vi "DialogCreateClass.vi"(0 "ClassWriterNative.lvclass":refnum<class "ClassWriterNative.lvclass">, 1 "ProjectItem Refnum":refnum<vi>, 5 "error in (no error)":errorcluster) -> (13 "InterfaceToImplement":T5, 14 "Reference out":refnum<class "ClassWriterNative.lvclass">, 15 "Cancelled":bool, 16 "CreateClassData":T6, 17 "DesignPatternsToAddAfterCreation":string[](array[string]), 18 "ChangeProviderRequested":string, 19 "error out":errorcluster)   [LabVIEW 2020, in "ClassWriterNative.lvclass"]
uses:
  <resource>/Framework/Providers/Open_GDS/ClassProviders/Provider_LvNativeClass/ClassWriterNative_class/ClassWriterNative.lvclass
  C:/Program Files (x86)/National Instruments/LabVIEW 2020/resource/Framework/Providers/Open_GDS/ClassProviders/Provider_BaseClassInterface/ClassWriter_class/ClassWriter.lvclass
  <resource>/Framework/Providers/Open_GDS/ClassProviders/Provider_BaseClassInterface/CreateClassData.ctl
  <resource>/Framework/Providers/Open_GDS/ClassProviders/Provider_BaseClassInterface/ClassWriter_class/InterfacesToImplement.ctl
  <resource>/Framework/Providers/Open_GDS/ClassProviders/Common/ScriptingFunctions/Scripting_ConnectorPanePatternType.ctl
  <resource>/Framework/Providers/Open_GDS/ClassProviders/Provider_BaseClassInterface/BaseProvider_SubVIs/BaseProvider_WireList.ctl
  <resource>/Framework/Providers/Open_GDS/ClassProviders/Provider_BaseClassInterface/BaseProvider_SubVIs/BaseProvider_WireStyleType.ctl
  <resource>/Framework/Providers/Open_GDS/ClassProviders/Provider_BaseClassInterface/ClassTemplateType.ctl
  <resource>/Framework/Providers/Open_GDS/ClassProviders/Common/InterfaceLibrary/InterfaceInfo.ctl
  <resource>/Framework/Providers/Open_GDS/ClassProviders/Common/LvClass_class/GDSLvClass_ClassMethodInfo.ctl
  <vilib>/Utility/miscctls.llb/LVRectTypeDef.ctl
  <vilib>/Utility/miscctls.llb/LVPositionTypeDef.ctl
  <resource>/Framework/Providers/Open_GDS/ClassProviders/Provider_EndevoGOOP400/EndevoG4ProviderName.ctl
  <vilib>/Utility/miscctls.llb/LVPointTypeDef.ctl
  <vilib>/Utility/miscctls.llb/LVNodeAndColumnTypeDef.ctl
  <vilib>/picture/picture.llb/imagedata.ctl
  <vilib>/Utility/miscctls.llb/LVRowAndColumnUnsignedTypeDef.ctl
  5375c306-5cef-40a8-bf77-a54f91188c9c.vi
  <resource>/Framework/Providers/Open_GDS/ClassProviders/Provider_BaseClassInterface/ClassWriter_class/ClassWriter.lvclass
  <resource>/Framework/Providers/Open_GDS/ClassProviders/Common/InterfaceLibrary/InterfaceLibrary.lvlib
panel:
  in  "WireSelectionList":T1
  out "IconSelection":picture
  in  "ModifyProviders":bool
  in  "Help":bool
  in  "_ShowContextHelp":bool
  out "Icon":picture
  in  "ConnectorPanePattern":T3 caption="Connector Pane" items=["4x4x4", "5x6x5", "6x8x6"]
  in  "ModifyTemplates":bool
  in  "AddDesignPattern":bool caption="DESIGN PATTERN"
  out "ProductPicture":picture
  out "TriggerSuffixChange":string
  in  "_CurrentClassProvider":u16(ring) caption="Class Provider To Use" items=["By Reference DVR (GOOP4)", "LVClass by value", "By Reference (GOOP3)"]
  in  "_UseLLB":bool
  out "DupPath":bool
  in  "_ClassType":i32(listbox) caption="Class Templates"
  in  "_ClassFolderSuffix":string caption="Folder Suffix"
  in  "_ClassName":string caption="Class Name"
  in  "_ClassDescription":string caption="Class Description"
  in  "_ClassFolder":path caption="Save Class To.."
  out "Wire Style":cluster{"Name":string, "Wire":picture}
  in  "ParentClassFilter":string caption="Filter"
  in  "_SelectParentClass":string(tree)="Derived Class" caption="Select Parent Class"
  in  "CreateInterfaceMethods":T4(ring)
  in  "InterfaceFilter":string caption="Filter"
  in  "_SelectInterfaceClass":i32[](listbox) caption="Select Parent Interface(s) (ctrl+click to do multiple Selection)"
  in  "_Cancel":bool
  in  "_CreateClass":bool
  out "DesignPatternDescription":string caption="Design Pattern Description"
  in  "DesignPatternList":i32(listbox) caption="Design Patterns"
  # "DESIGN PATTERNS SELECTION"
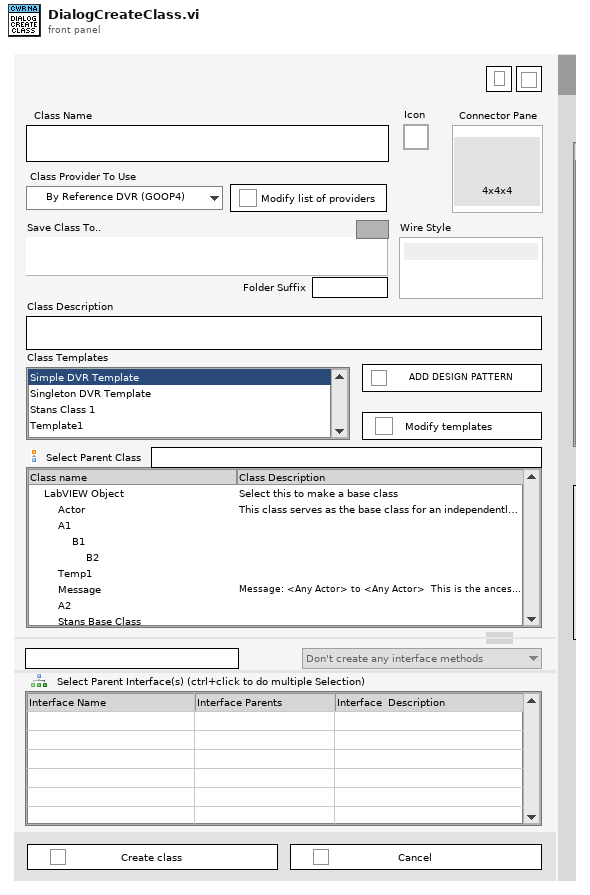
[diagram p1: front panel]
types:
  T1 = typedef "BaseProvider_WireList.ctl" = cluster{"WireStyle":T2[], "WireEditor":bool}
  T2 = typedef "BaseProvider_WireStyleType.ctl" = cluster{"Boolean":bool, "Wire":picture, "Name":string, "Status":u16}
  T3 = typedef "Scripting_ConnectorPanePatternType.ctl" = u16
  T4 = enum16{"Don't create any interface methods", "Create some interface methods", "Create all interface methods"}
  T5 = typedef "ClassWriter.lvclass/InterfacesToImplement.ctl" = cluster{"InterfacePath":path[], "CreateMethods":bool, "MethodsPerInterface(Empty=>All)":cluster{"Methods":string[]}[]}
  T6 = typedef "ClassWriter.lvclass/CreateClassData.ctl" = cluster{"ClassName":string, "ClassFolder":path, "ClassDescription":string, "ClassTemplateOptions":string, "BaseClass(ProjectStringPath or LvClassFilePath)":variant, "ExtraCreateParameters":variant, "FolderSuffix":string, "ParentInterfaces":path[]}
  T7 = cluster{"Font Name":string, "Size":u16, "Bold":bool, "Italic":bool, "Underline":bool, "Strikeout":bool, "Color":u32}
  T8 = typedef "LVPositionTypeDef.ctl" = cluster{"Left":i32, "Top":i32}
  T9 = typedef "LVRectTypeDef.ctl" = cluster{"Left":i16, "Top":i16, "Right":i16, "Bottom":i16}
  T10 = typedef "ClassWriter.lvclass/ClassTemplateType.ctl" = cluster{"TemplateIdName":string, "TemplateUserDialogName":string, "OnlySubClassTemplate":bool, "CanDeriveFromTheseTemplateIDs":string[], "ClassSuffix":string, "Description":string, "LvLibTemplate":bool, "CustomLocation":path}
  T11 = typedef "InterfaceLibrary.lvlib/InterfaceInfo.ctl" = cluster{"Name(Short if no Conflicts)":string, "FullQualifierName":string, "Description":string, "Path":path, "ParentInterfaceNames(Short if no Conflitcs)":string[], "ParentInterfaceFullQualifierNames":string[], "IconPath":path, "Methods":T12[], "DynamicDispatchMethod":bool[]}
  T12 = typedef "GDSLvClass_ClassMethodInfo.ctl" = cluster{"Name":string, "Descriptions":string, "RelativePath":path, "SourceScope":enum32{"invalid scope", "public", "private", "protected", "community"}, "MustOverride":bool, "VirtualFolderLocation":string[], "DynamicDispatch":bool}
  T13 = cluster{"Cancel":bool, "OtherTemplates":string[], "BaseClasses":path[], "Templates":T10[], "BaseObjectTag":string, "ClassType(Template)":string, "BaseClassToUse":path, "DeriveFromClass":path, "OpenG":bool, "Derived":bool, "DeriveFromClassRef":refnum<vi>, "ClassPaths":path[], "DesignPatternsVisible":bool, "ClassProviderName":string, "ClassTemplateUsed":string, "PlugInIDs":string[], "DPDescriptions":string[], "DpDependencies":cluster{"DependenciesID":string[]}[], "DPs":string[], "InitDerived":bool, "ClassFolderSuffix":string, "ChangeProviderTo":string, "ClassTags":string[], "LLB_Allowed":bool, "StartFolder":path, "SplitterMouseDown":bool, "InterfaceIcons":path[], "InterfaceInfo":T11[], "OldBnds":T9, "BondsChanged":bool, "ClassTemplateIndex":i32[], "StartBnds":T9, "StartInterfacePath":path, "Providers":string[], "LastProvderValues":cluster{"_ClassName":string, "_ClassFolder":path, "_ClassDescription":string, "Created":timestamp}, "ParentInterfaces":path[], "InterfacesInList":path[]}
  T14 = typedef "EndevoG4ProviderName.ctl" = enum16{"EndevoGOOP400"}
  T15 = typedef "LVPointTypeDef.ctl" = cluster{"Horizontal":i16, "Vertical":i16}
  T16 = typedef "LVNodeAndColumnTypeDef.ctl" = cluster{"Node":string, "Column":i32}
  T17 = typedef "imagedata.ctl" = cluster{"image type":i32, "image depth":i32, "image":u8[], "mask":u8[], "colors":u32[], "Rectangle":cluster{"left":i16, "top":i16, "right":i16, "bottom":i16}}
  T18 = typedef "LVRowAndColumnUnsignedTypeDef.ctl" = cluster{"Row":u32, "Column":u32}
  T19 = enum8{"Enabled", "Disabled", "Disabled and Grayed Out"}
  T20 = cluster{"_ClassName":string, "_ClassFolder":path, "_ClassDescription":string, "seconds since 1Jan1904":timestamp}
  T21 = typedef "GDSLvCLass_ClassSettingsType.ctl" = cluster{"ClassProviderName":string, "ClassTemplateUsed":string, "ClassTemplateVersion":string, "ClassDescription":string, "PlugIns":T22[], "ConnectorPanePattern":string}
  T22 = typedef "GDSLvClass_PlugIn.ctl" = cluster{"Type":T23, "ID":string, "Version":string, "Path":path, "Name":string, "Data":variant}
  T23 = typedef "GDSLvClass_PlugInTypes.ctl" = enum16{"DesignPattern", "MethodTypes"}
  T24 = typedef "BaseProvider_IniFileSettings.ctl" = cluster{"ClassFolderSuffix":string, "InterfaceFolderSuffix":string, "InterfaceIcon":string, "FileNamingOption":T25, "DynamicDispatchStartValue":bool, "UseGetSetForPropertyNodeMethods":bool}
  T25 = typedef "BaseProvider_FileNamingOption.ctl" = enum16{"CamelCase", "Space", "Underscore"}
  T26 = enum32{"Invalid", "Standard", "Closed", "Hidden", "Minimized", "Maximized"}
  T27 = cluster{"_ClassName":string, "_ClassFolder":path, "_ClassDescription":string, "Created":timestamp}
  T28 = typedef "GOOP_WireConfigurationType.ctl" = cluster{"Edge thickness":i32, "Edge color":u32, "Center thickness":i32, "Center pattern":T29, "CenterColor1":u32, "CenterColor2":u32, "Tunnels and terminals colors":u32}
  T29 = typedef "GOOP_WirePattern.ctl" = enum16{"Solid", "Large dash", "Small dash"}
  T30 = typedef "LVPoint32TypeDef.ctl" = cluster{"Horizontal":i32, "Vertical":i32}
  T31 = typedef "DesignPatternsData.ctl" = cluster{"Type":string, "Patterns":cluster{"ID":string, "Path":path, "Name":string, "Desc":string, "Version":string, "DependenciesID":string[], "OnlyOne":bool}[]}
  T32 = cluster{"ID":string, "Path":path, "Name":string, "Desc":string, "Version":string, "DependenciesID":string[], "OnlyOne":bool}[]
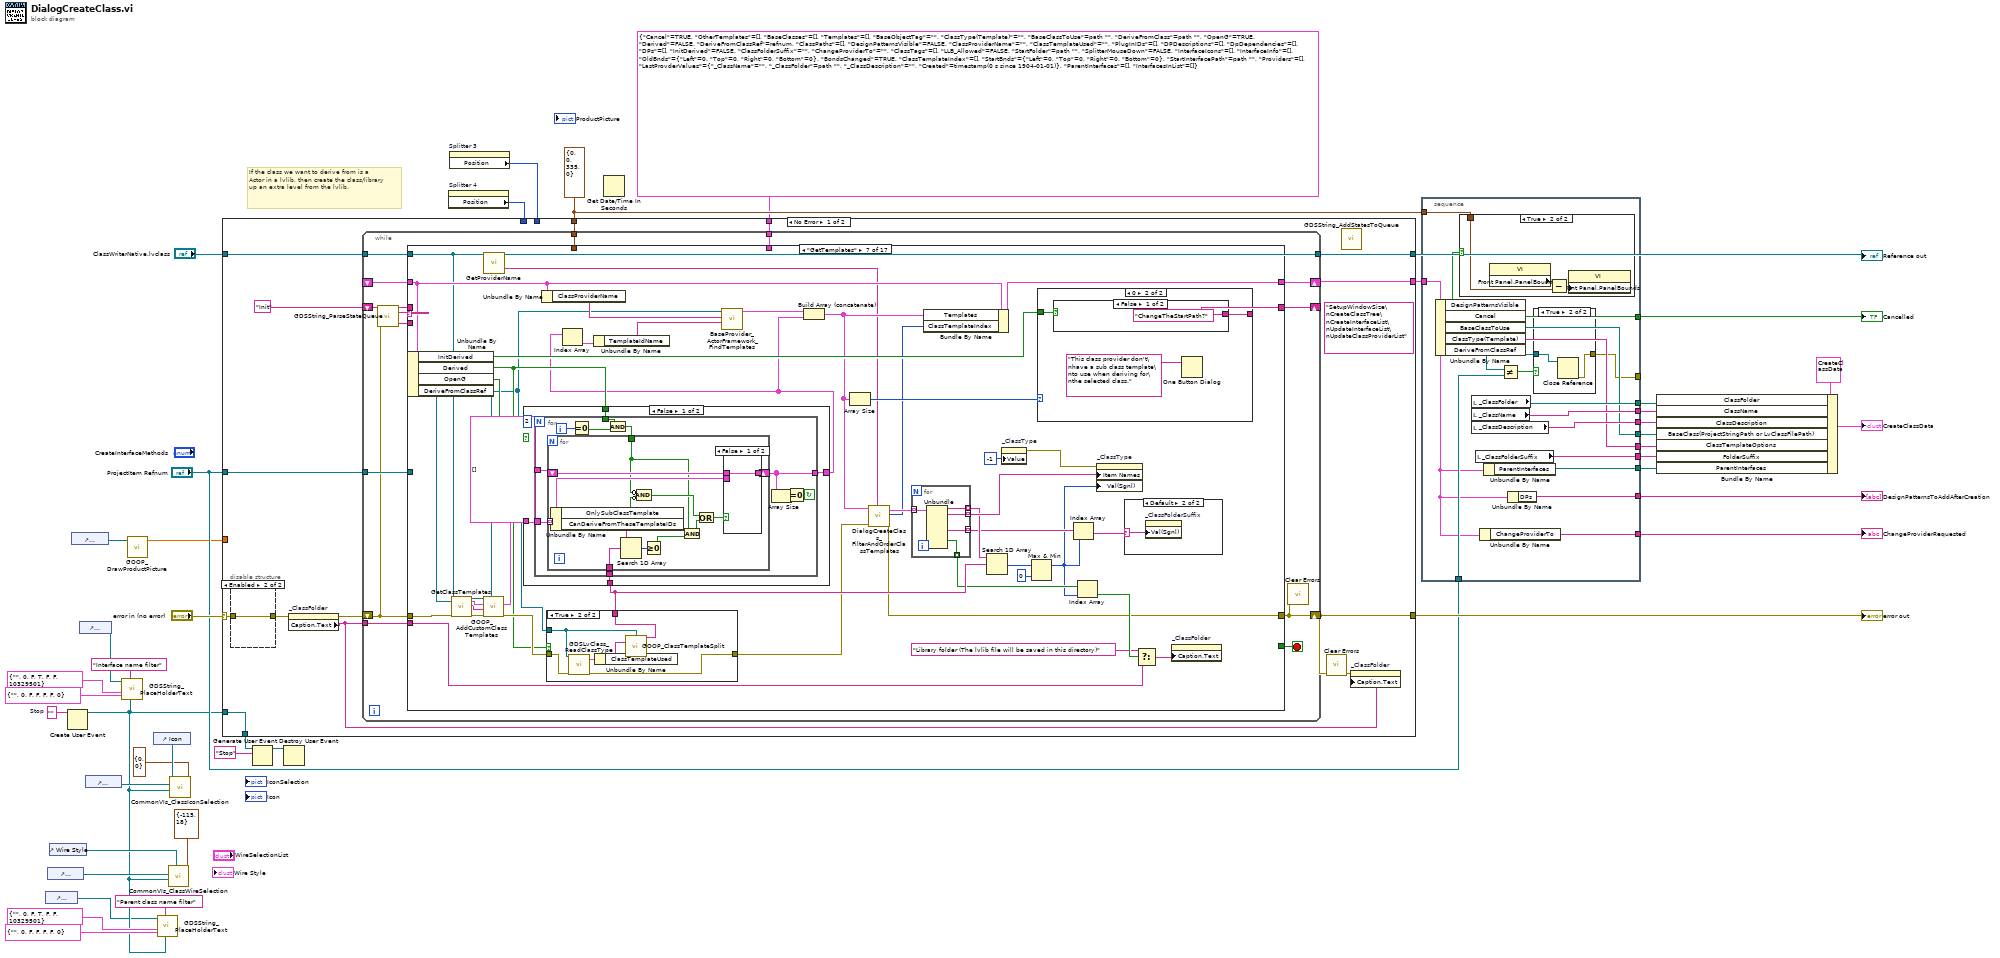
[diagram p0: block diagram]
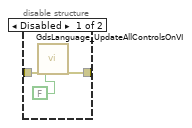
[diagram p4: hidden frame]
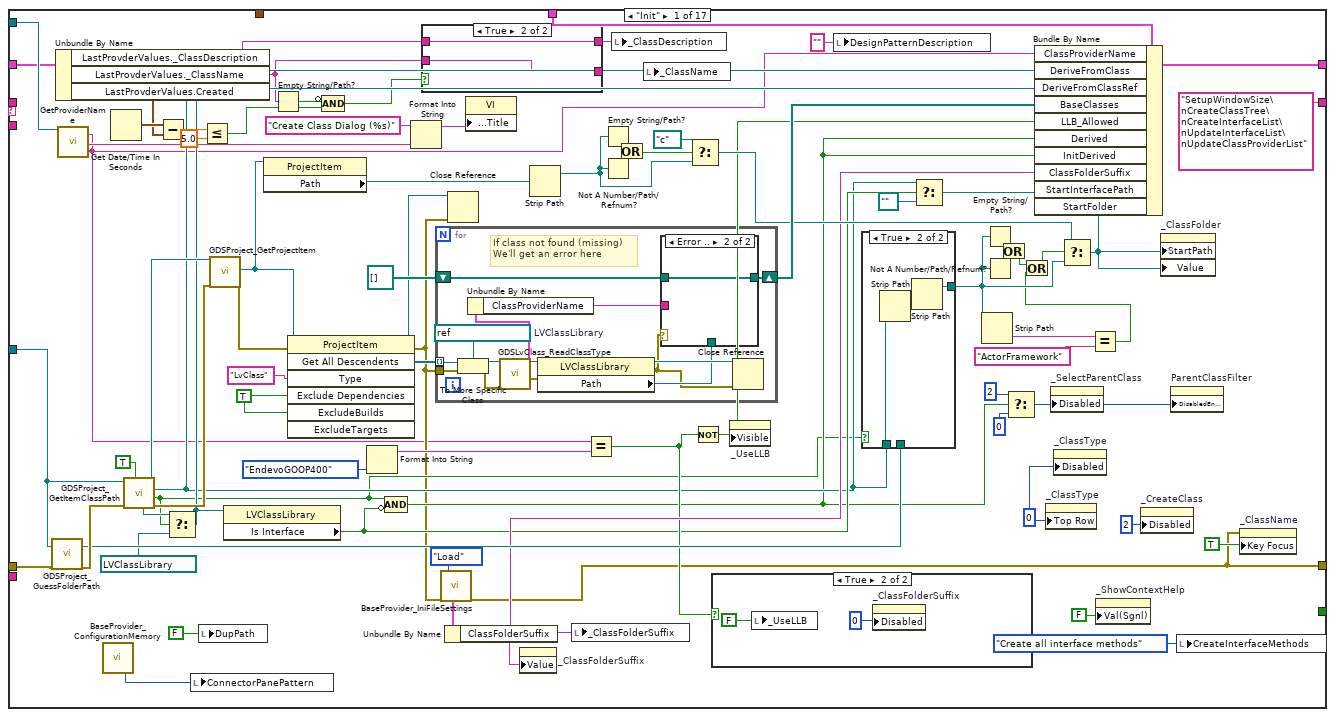
[diagram p5: hidden frame]
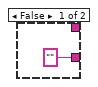
[diagram p6: hidden frame]
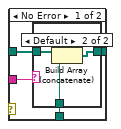
[diagram p8: hidden frame]
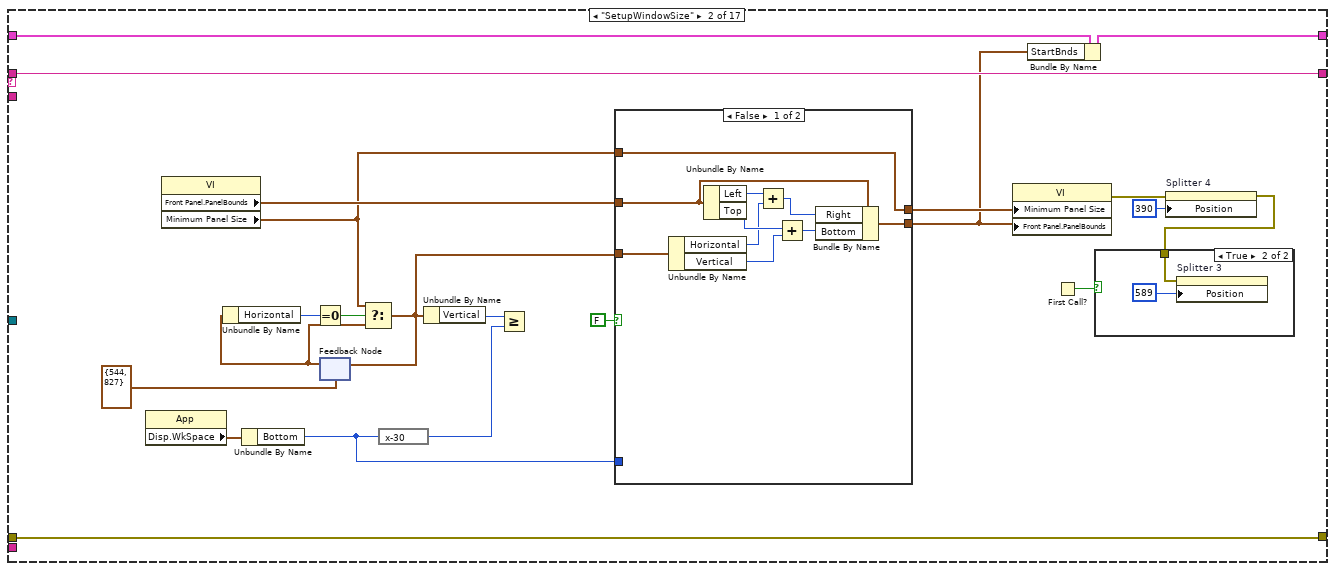
[diagram p11: hidden frame]
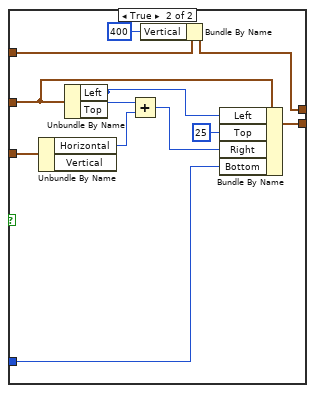
[diagram p13: hidden frame]
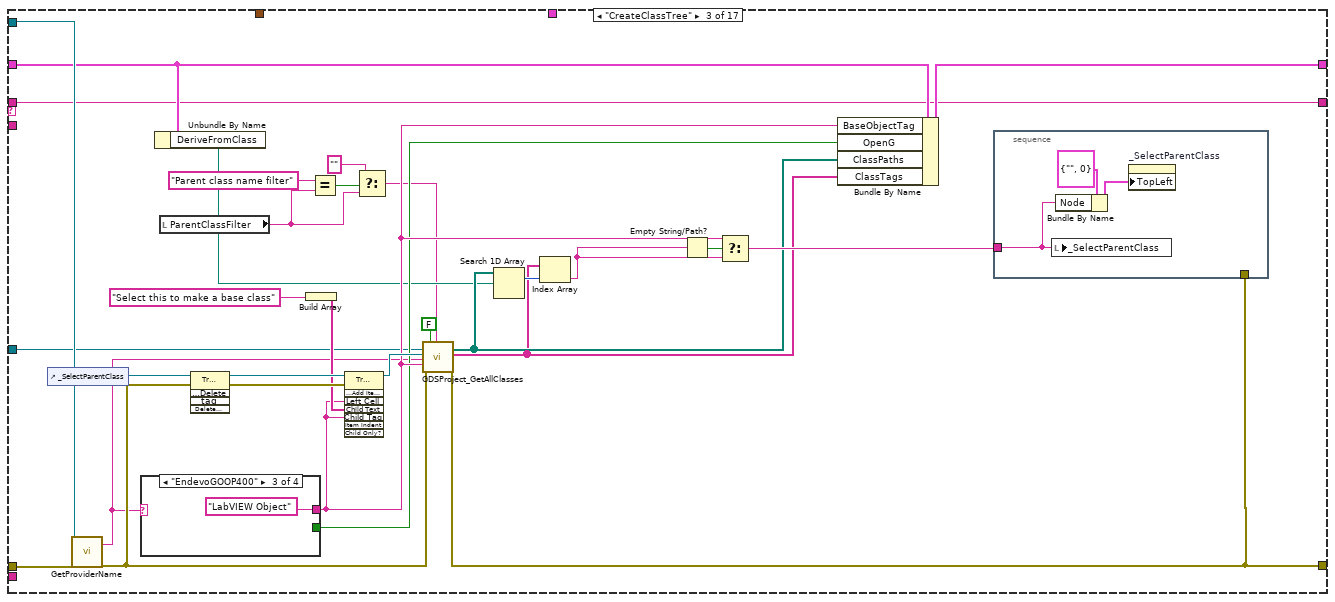
[diagram p14: hidden frame]
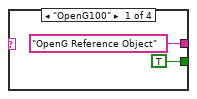
[diagram p15: hidden frame]
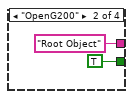
[diagram p16: hidden frame]
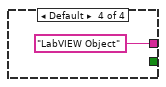
[diagram p17: hidden frame]
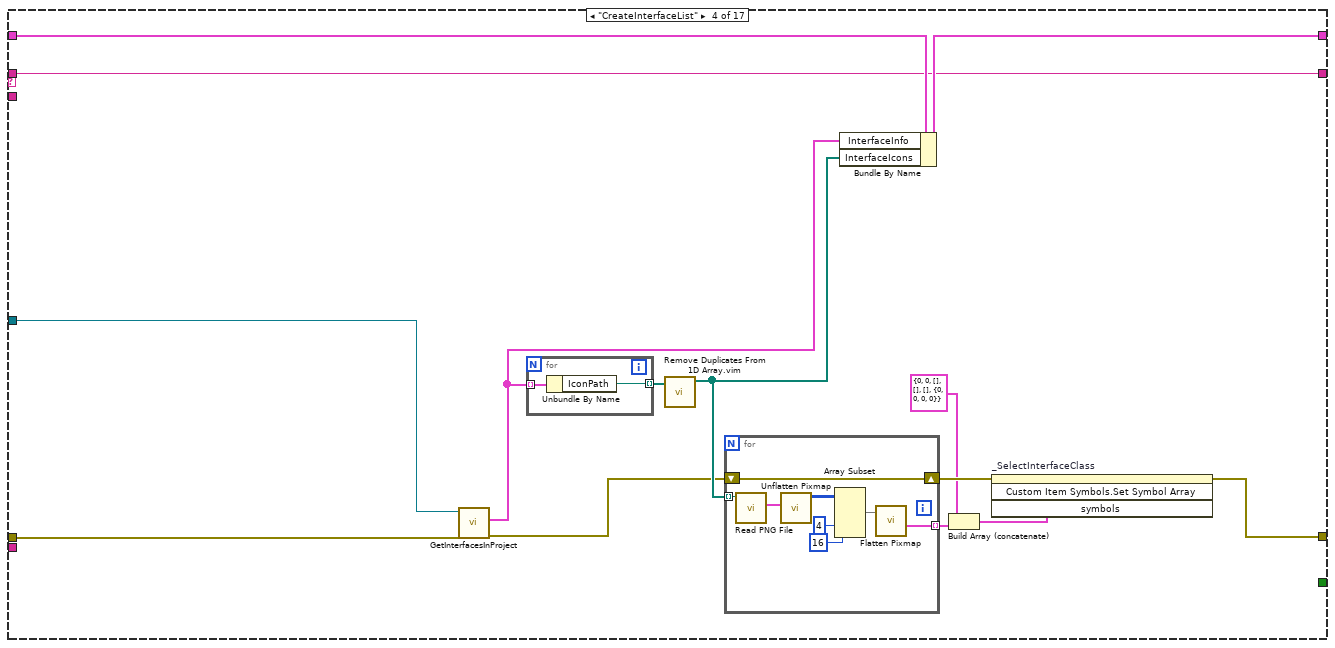
[diagram p18: hidden frame]
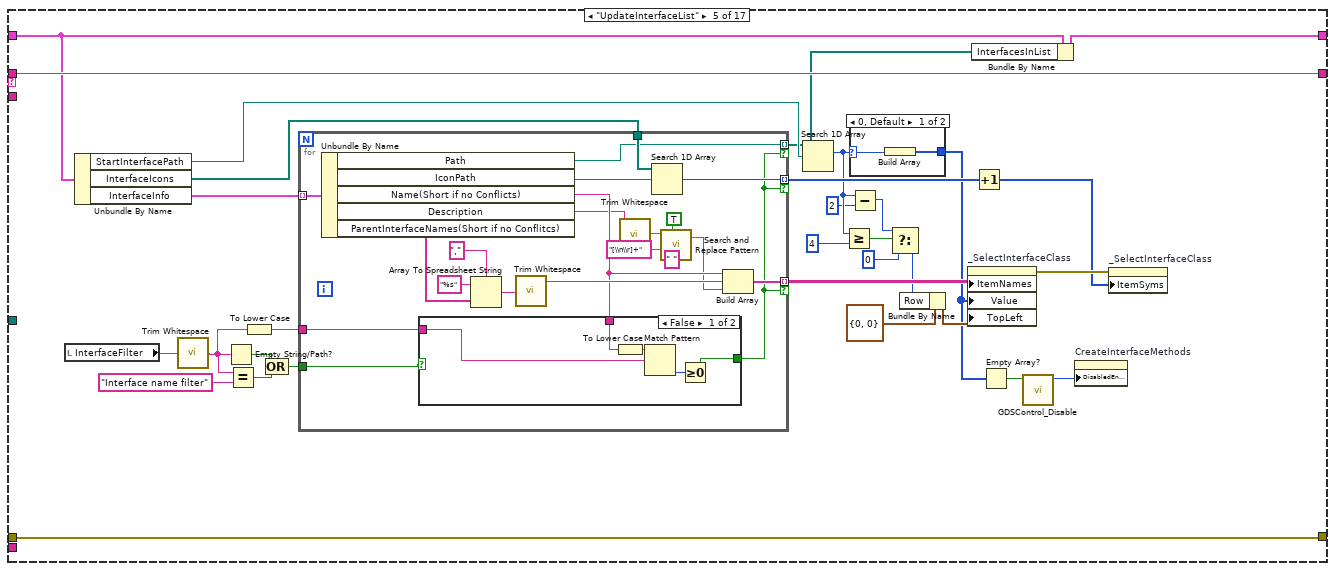
[diagram p19: hidden frame]
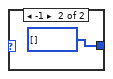
[diagram p20: hidden frame]
diagram:
  w16 = ""  # Stop
  w29 = T9 {"Left"=0, "Top"=0, "Right"=335, "Bottom"=0} ("Rect")
  # "If the class we want to derive from is a\nActor in a lvlib, then create the class/library\nup an extra level from the lvlib."
  n1 = control-ref of="ParentClassFilter"() -> (w1:refnum<vi>)
  n2 = control-ref of="WireSelectionList"() -> (w10:refnum<vi>)
  n3 = control-ref of="Wire Style"() -> (w9:refnum<vi>)
  n4 = Create User Event(user event datatype=w16) -> (user event=w2:refnum<user-event>)  [unwired: 1 in, 1 out]
  n5 = control-ref of="ProductPicture"() -> (w25:refnum<vi>)
  n6 = control-ref of="InterfaceFilter"() -> (w23:refnum<vi>)
  n7 = control-ref of="IconSelection"() -> (w17:refnum<vi>)
  n8 = call <resource>:"GDSString_PlaceHolderText.vi"("BooleanUserEventToStopPlaceHolderVI"=w2, "PlaceholderText"="Interface name filter" ("InterfaceFilter"), "PlaceholderTextFont(Grey,Italic)"=T7 {"Font Name"="", "Size"=0, "Bold"=FALSE, "Italic"=TRUE, "Underline"=FALSE, "Strikeout"=FALSE, "Color"=10329501}, "NormalTextFont(Black)"=T7 {"Font Name"="", "Size"=0, "Bold"=FALSE, "Italic"=FALSE, "Underline"=FALSE, "Strikeout"=FALSE, "Color"=0}, "PlaceholderStringRef"=w23) -> ()  [unwired: 6 in, 1 out]
  n9 = call <resource>:"GOOP_DrawProductPicture.vi"("ProductPictureControl"=w25) -> ("Zoom Factor"=w24:sgl)  [unwired: 10 in]
  n10 = control-ref of="Icon"() -> (w18:refnum<vi>)
  n11 = call <resource>:"GDSString_PlaceHolderText.vi"("BooleanUserEventToStopPlaceHolderVI"=w2, "PlaceholderText"="Parent class name filter" ("InterfaceFilter"), "PlaceholderTextFont(Grey,Italic)"=T7 {"Font Name"="", "Size"=0, "Bold"=FALSE, "Italic"=TRUE, "Underline"=FALSE, "Strikeout"=FALSE, "Color"=10329501}, "NormalTextFont(Black)"=T7 {"Font Name"="", "Size"=0, "Bold"=FALSE, "Italic"=FALSE, "Underline"=FALSE, "Strikeout"=FALSE, "Color"=0}, "PlaceholderStringRef"=w1) -> ()  [unwired: 6 in, 1 out]
  n12 = call <resource>:"CommonVIs_ClassWireSelection.vi"("Offset(-300,0)"=T8 {"Left"=-115, "Top"=18}, "SelectedWireStyle"=w9, "Messages(Stop or Empty string will stop this VI)"=w2, "WireSelectionList"=w10) -> ()  [unwired: 7 in, 1 out]
  n13 = call <resource>:"CommonVIs_ClassIconSelection.vi"("Offset"=T8 {"Left"=0, "Top"=0}, "Icon"=w18, "Messages(Stop or Empty string will stop this VI)"=w2, "IconSelection"=w17) -> ()  [unwired: 8 in]
  n14 = property on="Splitter 4" class="Splitter"() -> ("Position"=w13:i32)  [unwired: 2 in, 2 out]
  n15 = property on="Splitter 3" class="Splitter"() -> ("Position"=w12:i32)  [unwired: 2 in, 2 out]
  n16 = case shown="No Error" "error in (no error)" {
    selector: "error in (no error)" -> [w52 w1129]
    tunnel: "ClassWriterNative.lvclass" -> [w56 w1128]
    tunnel: [w45 w1129] -> w42
    tunnel: [w57 w1128] -> w40
    tunnel: T13 {"Cancel"=TRUE, "OtherTemplates"=[], "BaseClasses"=[], "Templates"=[], "BaseObjectTag"="", "ClassType(Template)"="", "BaseClassToUse"=path "", "DeriveFromClass"=path "", "OpenG"=TRUE, "Derived"=FALSE, "DeriveFromClassRef"=refnum, "ClassPaths"=[], "DesignPatternsVisible"=FALSE, "ClassProviderName"="", "ClassTemplateUsed"="", "PlugInIDs"=[], "DPDescriptions"=[], "DpDependencies"=[], "DPs"=[], "InitDerived"=FALSE, "ClassFolderSuffix"="", "ChangeProviderTo"="", "ClassTags"=[], "LLB_Allowed"=FALSE, "StartFolder"=path "", "SplitterMouseDown"=FALSE, "InterfaceIcons"=[], "InterfaceInfo"=[], "OldBnds"={"Left"=0, "Top"=0, "Right"=0, "Bottom"=0}, "BondsChanged"=TRUE, "ClassTemplateIndex"=[], "StartBnds"={"Left"=0, "Top"=0, "Right"=0, "Bottom"=0}, "StartInterfacePath"=path "", "Providers"=[], "LastProvderValues"={"_ClassName"="", "_ClassFolder"=path "", "_ClassDescription"="", "Created"=timestamp(0 s since 1904-01-01)}, "ParentInterfaces"=[], "InterfacesInList"=[]} ("output cluster") -> [w55 _]
    tunnel: "ProjectItem Refnum" -> [w54 _]
    tunnel: [w53 _] -> w39
    tunnel: w29 -> [w51 _]
    tunnel: w24 -> [_ _]
    tunnel: w2 -> [w47 w1127]
    tunnel: [w47 w1127] -> w20
    tunnel: w13 -> [_ _]
    tunnel: w12 -> [_ _]
    frame No Error {
      (unwired) "SetupWindowSize\nCreateClassTree\nCreateInterfaceList\nUpdateInterfaceList\nUpdateClassProviderList"
      n17 = disable-structure shown="Enabled" {
        disable-tunnel: w52 -> [w60 w61]
        disable-tunnel: [w58 w61] -> w50
        frame Disabled {
          n18 = call <resource>:"GdsLanguage_UpdateAllControlsOnVI.vi"("error in (no error)"=w60, "CreateLanguageFile(Use this to create a languageFile)"=FALSE) -> ("error out"=w58:errorcluster)  [unwired: 16 in, 1 out]
        }
        frame Enabled {
        }
      }
      n19 = property on="_ClassFolder" class="Path"(error in=w50) -> (error out=w49:errorcluster, "Caption.Text"=w48:string)  [unwired: 1 in, 1 out]
      n20 = while {
        shift-right: [w62] -> w45
        shift-left: w49 -> [w68]
        shift-right: [w66] -> _
        shift-left: "Init" -> [w69]
        shift-right: [w72] -> w53
        shift-left: _ -> [w76]
        tunnel: w56 -> [w75]
        tunnel: [w75] -> w57
        tunnel: w55 -> [w74]
        tunnel: w54 -> [w73]
        tunnel: w51 -> [w71]
        tunnel: w48 -> [w70]
        stop <- w67 stop-if-true
        n21 = call <resource>:"GDSString_ParseStateQueue.vi"("State Queue"=w69, "Error In (no error)"=w68) -> ("Remaining States"=w64:string, "Current State"=w65:string, "Arguments"=w63:string)  [unwired: 9 in, 2 out]
        n22 = case shown="\"GetTemplates\"" w65 {
          tunnel: w76 -> [w92 w209 w253 w284 w324 w366 w405 w483 w509 w518 w914 w928 w957 w1018 w1096 w1122 w1126]
          tunnel: [w154 w193 w255 w285 w300 w365 w421 w483 w509 w538 w915 w943 w956 w1045 w1096 w1122 w1126] -> w72
          tunnel: w68 -> [w134 w208 w258 w272 w325 w372 w418 w479 w508 w541 w919 w945 w966 w1036 w1102 _ w1125]
          tunnel: [w80 w208 w238 w276 w325 w372 w390 w479 w508 w541 w919 w945 w965 w1035 w1102 errorcluster {"status"=TRUE, "code"=1, "source"="Invalid Case"} ("error out") w1125] -> w62
          tunnel: w75 -> [w127 _ w261 _ _ w367 w383 _ _ w511 _ w921 _ _ _ _ _]
          tunnel: ["SetupWindowSize\nCreateClassTree\nCreateInterfaceList\nUpdateInterfaceList\nUpdateClassProviderList" w207 w239 w273 w326 "GetTemplates" w422 "Idle" "Idle" w539 w918 w944 "Idle" "GetInterfaceSettings" "Exit" "Exit" "Exit"] -> w66
          tunnel: w74 -> [w153 _ _ _ _ _ _ _ _ _ _ _ _ _ _ _ _]
          tunnel: w73 -> [w132 _ w240 w283 _ _ _ _ _ w523 _ _ _ _ _ _ _]
          tunnel: w71 -> [_ _ _ _ _ _ _ _ _ w521 _ _ _ _ _ _ _]
          tunnel: w70 -> [_ _ _ _ _ _ w398 _ _ w520 _ w930 _ _ _ _ _]
          tunnel: [_ _ _ _ _ _ _ _ _ _ _ _ _ _ _ TRUE TRUE] -> w67
          tunnel: w64 -> [_ w207 w239 w273 w326 _ _ _ _ _ w918 w944 _ _ _ _ _]
          tunnel: w63 -> [_ _ _ _ _ _ _ _ _ _ _ _ _ _ _ _ _]
          frame "Init" {
            w123 = 0 ("Top Row")
            w126 = TRUE ("ExcludeDependencies")
            n23 = call <resource>:"GDSProject_GuessFolderPath.vi"("ProjectItem"=w132, "error in (no error)"=w134) -> ("Path"=w131:path, "error out"=w133:errorcluster)  [unwired: 14 in, 2 out]
            n24 = Unbundle By Name(w92) -> ("LastProvderValues._ClassDescription"=w84:string, "LastProvderValues._ClassName"=w85:string, "LastProvderValues.Created"=w90:timestamp)
            n25 = call-dynamic "GetProviderName.vi"("ClassWriterNative in"=w127) -> ("ProviderName"=w78:string, "TranslatedProviderName"=w79:string)  [unwired: 14 in, 3 out]
            n26 = call <resource>:"BaseProvider_ConfigurationMemory.vi"() -> ("PatternOut"=w103:T3)  [unwired: 13 in, 6 out]
            n27 = Get Date/Time In Seconds() -> (seconds since 1Jan1904=w91:timestamp)
            n28 = call <resource>:"GDSProject_GetItemClassPath.vi"("ReturnRefToClass(False)"=TRUE, "error in"=w133, "ProjectItemRefIn"=w132) -> ("error out"=w150:errorcluster, "LvCLassFound"=w93:bool, "Path"=w99:path, "ProjectItemRefOut"=w148:refnum<vi>, "LvClassRef"=w122:refnum<vi>)  [unwired: 3 in, 1 out]
            n29 = Subtract(x=w91, y=w90) -> (x-y=w89:dbl)
            n30 = Select(t=w122, s=w93, f=refnum<vi> refnum) -> (s? t:f=w101:refnum<vi>)
            n31 = local write "ConnectorPanePattern"(w103) -> ()
            n32 = local write "DupPath"(FALSE ("DupPath")) -> ()
            n33 = Less Or Equal?(x=w89, y=5.0) -> (x <= y?=w86:bool)
            n34 = call <resource>:"GDSProject_GetProjectItem.vi"("ProjectItemToSearchFrom"=w148, "error in (no error)"=w150) -> ("ProjectItemFound"=w102:refnum<vi>, "error out"=w149:errorcluster)  [unwired: 14 in, 2 out]
            n35 = property class="LVClassLibrary"(reference=w101) -> ("Is Interface"=w100:bool)  [unwired: 1 in, 2 out]
            n36 = property class="ProjectItem"(reference=w102) -> ("Path"=w136:path)  [unwired: 1 in, 2 out]
            n37 = Empty String/Path?(string/path=w85) -> (empty?=w87:bool)
            n38 = invoke class="ProjectItem" method="Get All Descendents"(reference=w102, error in=w149, "Type"="LvClass" ("x"), "Exclude Dependencies"=w126, "ExcludeBuilds"=w126) -> (reference out=w145:refnum<vi>, error out=w80:errorcluster, "All Descendents"=w147:refnum<vi>[])  [unwired: 2 in, 4 out]
            n39 = Compound Arithmetic op=AND(invert w87, w86) -> (w83:bool)
            n40 = Format Into String(EndevoG4ProviderName."EndevoGOOP400" ("ProviderName")) -> (resulting string=w118:string)  [unwired: 3 in, 1 out]
            n41 = Compound Arithmetic op=AND(w93, invert w100) -> (w96:bool)
            n42 = Format Into String(format string="Create Class Dialog (%s)", w79) -> (resulting string=w129:string)  [unwired: 2 in, 1 out]
            n43 = case shown="True" w83 {
              tunnel: w85 -> [_ w157]
              tunnel: w84 -> [_ w158]
              tunnel: [_ w158] -> w82
              tunnel: ["" ("Class name") w157] -> w81
              frame False {
              }
              frame True {
              }
            }
            n44 = for {
              tunnel: w147 -> [w174] mode=indexing
              shift-right: [w170] -> w144
              shift-left: path[] [] -> [w169]
              tunnel: w80 -> [w166]
              w173 = refnum<vi> refnum  # LVClassLibrary
              # "If class not found (missing)\nWe'll get an error here"
              n45 = To More Specific Class(target class=w173, reference=w174, error in=w166) -> (specific class reference=w172:refnum<vi>, error out=w171:errorcluster)
              n46 = call <resource>:"GDSLvClass_ReadClassType.vi"("Class Refnum In"=w172, "error in (no error)"=w171) -> ("Class Refnum Out"=w167:refnum<vi>, "ClassSettings"=w165:T21, "error out"=w168:errorcluster)  [unwired: 15 in]
              n47 = Unbundle By Name(w165) -> ("ClassProviderName"=w164:string)
              n48 = property class="LVClassLibrary"(reference=w167, error in=w168) -> (reference out=w163:refnum<vi>, error out=w161:errorcluster, "Path"=w162:path)
              n49 = case shown="Error .." w161 {
                tunnel: [w178 w183] -> w170
                tunnel: w169 -> [w177 w183]
                tunnel: w164 -> [w176 _]
                tunnel: w162 -> [w175 _]
                frame No Error {
                  n50 = case shown="Default" w176 {
                    tunnel: [w179 w182] -> w178
                    tunnel: w177 -> [w179 w181]
                    tunnel: w175 -> [_ w180]
                    frame "" {
                    }
                    frame Default {
                      n51 = Build Array (concatenate)(w181, w180) -> (w182:path[])
                    }
                  }
                }
                frame Error {
                }
              }
              n52 = Close Reference(reference=w163, error in (no error)=w161) -> ()  [unwired: 1 out]
            }
            n53 = call <resource>:"BaseProvider_IniFileSettings.vi"("error in (no error)"=w80, "Action"=enum16{"Read", "Load", "Save"}."Load") -> ("IniFileSettings"=w116:T24)  [unwired: 16 in, 1 out]
            n54 = Unbundle By Name(w116) -> ("ClassFolderSuffix"=w115:string)
            n55 = Close Reference(reference=w145, error in (no error)=w80) -> ()  [unwired: 1 out]
            n56 = property class="VI"("Front Panel.Title"=w129) -> ()  [unwired: 2 in, 2 out]
            n57 = property on="_ClassFolderSuffix" class="Str"("Value"=w115) -> ()  [unwired: 2 in, 2 out]
            n58 = Strip Path(path=w136) -> (stripped path=w135:path)  [unwired: 1 out]
            n59 = local write "_ClassFolderSuffix"(w115) -> ()
            n60 = Equal?(x=w78, y=w118) -> (x = y?=w113:bool)
            n61 = Empty String/Path?(string/path=w135) -> (empty?=w137:bool)
            n62 = Not A Number/Path/Refnum?(number/path/refnum=w135) -> (NaN/Path/Refnum?=w138:bool)
            n63 = local write "_ClassDescription"(w82) -> ()
            n64 = Or(x=w137, y=w138) -> (x .or. y?=w139:bool)
            n65 = local write "_ClassName"(w81) -> ()
            n66 = Select(t=path "c:/", s=w139, f=w135) -> (s? t:f=w124:path)
            n67 = Not(x=w113) -> (.not. x?=w114:bool)
            n68 = case shown="True" w113 {
              frame False {
              }
              frame True {
                n69 = local write "_UseLLB"(FALSE ("_UseLLB")) -> ()
                n70 = property on="_ClassFolderSuffix" class="Str"("Disabled"=u8 0) -> ()  [unwired: 2 in, 2 out]
              }
            }
            n71 = property on="_UseLLB" class="Bool (strict)"("Visible"=w114) -> ()  [unwired: 2 in, 2 out]
            n72 = local write "DesignPatternDescription"("" ("DesignPatternDescription")) -> ()
            n73 = case shown="True" w93 {
              tunnel: w99 -> [_ w187]
              tunnel: [w184 w185] -> w111
              tunnel: w131 -> [w184 _]
              frame False {
              }
              frame True {
                n74 = Strip Path(path=w187) -> (stripped path=w186:path)  [unwired: 1 out]
                n75 = Strip Path(path=w186) -> (stripped path=w185:path)  [unwired: 1 out]
              }
            }
            n76 = Select(t=w99, s=w100, f=path "") -> (s? t:f=w97:path)
            n77 = Strip Path(path=w111) -> (name=w110:string)  [unwired: 1 out]
            n78 = Empty String/Path?(string/path=w111) -> (empty?=w142:bool)
            n79 = Not A Number/Path/Refnum?(number/path/refnum=w111) -> (NaN/Path/Refnum?=w141:bool)
            n80 = Or(x=w142, y=w141) -> (x .or. y?=w108:bool)
            n81 = Select(t=u8 2 ("Disabled"), s=w96, f=u8 0 ("Disabled")) -> (s? t:f=w77:u8)
            n82 = property on="_ClassType" class="LstBox (strict)"("Top Row"=w123) -> ()  [unwired: 2 in, 2 out]
            n83 = property on="_SelectParentClass" class="Tree (strict)"("Disabled"=w77) -> ()  [unwired: 2 in, 2 out]
            n84 = property on="_ClassType" class="LstBox (strict)"("Disabled"=w123) -> ()  [unwired: 2 in, 2 out]
            n85 = Equal?(x=w110, y="ActorFramework") -> (x = y?=w107:bool)
            n86 = Or(x=w108, y=w107) -> (x .or. y?=w106:bool)
            n87 = Select(t=w124, s=w106, f=w111) -> (s? t:f=w112:path)
            n88 = Bundle By Name(cluster=w153, "ClassProviderName"=w78, "DeriveFromClass"=w99, "DeriveFromClassRef"=w101, "BaseClasses"=w144, "LLB_Allowed"=w114, "Derived"=w96, "InitDerived"=w96, "ClassFolderSuffix"=w115, "StartInterfacePath"=w97, "StartFolder"=w112) -> (w154:T13)
            n89 = property on="_ShowContextHelp" class="Bool (strict)"("Val(Sgnl)"=FALSE ("Value (Signaling)")) -> ()  [unwired: 2 in, 2 out]
            n90 = property on="_CreateClass" class="Bool"("Disabled"=u8 2) -> ()  [unwired: 2 in, 2 out]
            n91 = property on="_ClassFolder" class="Path"("StartPath"=w112, "Value"=w112) -> ()  [unwired: 2 in, 2 out]
            n92 = property on="ParentClassFilter" class="Str"("DisabledEnum"=w77) -> ()  [unwired: 2 in, 2 out]
            n93 = local write "CreateInterfaceMethods"(T4."Create all interface methods" ("CreateInterfaceMethods")) -> ()
            n94 = property on="_ClassName" class="Str"(error in=w80, "Key Focus"=TRUE) -> ()  [unwired: 1 in, 2 out]
          }
          frame "SetupWindowSize" {
            n95 = property class="App"() -> ("Disp.WkSpace"=w206:T9)  [unwired: 2 in, 2 out]
            n96 = property class="VI"() -> ("Front Panel.PanelBounds"=w205:T9, "Minimum Panel Size"=w195:T15)  [unwired: 2 in, 2 out]
            n97 = Unbundle By Name(w206) -> ("Bottom"=w198:i16)
            n98 = feedback #1(T15 {"Horizontal"=544, "Vertical"=827} ("Minimum Panel Size")) -> (w202:T15)
            n99 = Unbundle By Name(w202) -> ("Horizontal"=w204:i16)
            n100 = Equal To 0?(x=w204) -> (x = 0?=w203:bool)
            n101 = Select(t=w195, s=w203, f=w202) -> (s? t:f=w201:T15)
            n102 = feedback-in #1(w201) -> ()
            n103 = expression code="x-30"(w198) -> (w199:i16)
            n104 = Unbundle By Name(w201) -> ("Vertical"=w200:i16)
            n105 = Greater Or Equal?(x=w200, y=w199) -> ()  [unwired: 1 out]
            n106 = case shown="False" FALSE {
              tunnel: w205 -> [w214 w229]
              tunnel: w201 -> [w217 w232]
              tunnel: [w213 w230] -> w192
              tunnel: w198 -> [_ w225]
              tunnel: [w212 w223] -> w196
              tunnel: w195 -> [w212 w224]
              frame False {
                n107 = Unbundle By Name(w217) -> ("Horizontal"=w219:i16, "Vertical"=w221:i16)
                n108 = Unbundle By Name(w214) -> ("Left"=w218:i16, "Top"=w220:i16)
                n109 = Add(x=w218, y=w219) -> (x+y=w216:i16)
                n110 = Add(x=w220, y=w221) -> (x+y=w215:i16)
                n111 = Bundle By Name(cluster=w214, "Right"=w216, "Bottom"=w215) -> (w213:T9)
              }
              frame True {
                n112 = Unbundle By Name(w232) -> ("Horizontal"=w231:i16)  [unwired: 1 out]
                n113 = Unbundle By Name(w229) -> ("Left"=w228:i16)  [unwired: 1 out]
                n114 = Add(x=w228, y=w231) -> (x+y=w227:i16)
                n115 = Bundle By Name(cluster=w224, "Vertical"=i16 400) -> (w223:T15)
                n116 = Bundle By Name(cluster=w229, "Left"=w228, "Top"=i16 25, "Right"=w227, "Bottom"=w225) -> (w230:T9)
              }
            }
            n117 = property class="VI"("Minimum Panel Size"=w196, "Front Panel.PanelBounds"=w192) -> (error out=w191:errorcluster)  [unwired: 2 in, 1 out]
            n118 = Bundle By Name(cluster=w209, "StartBnds"=w192) -> (w193:T13)
            n119 = First Call?() -> (First Call?: T/F=w188:bool)
            n120 = property on="Splitter 4" class="Splitter"(error in=w191, "Position"=390 ("Splitter Position")) -> (error out=w189:errorcluster)  [unwired: 1 in, 1 out]
            n121 = case shown="True" w188 {
              tunnel: w189 -> [_ w211]
              frame False {
              }
              frame True {
                n122 = property on="Splitter 3" class="Splitter"(error in=w211, "Position"=589 ("Splitter Position")) -> ()  [unwired: 1 in, 2 out]
              }
            }
          }
          frame "CreateClassTree" {
            n123 = control-ref of="_SelectParentClass"() -> (w262:refnum<vi>)
            n124 = call-dynamic "GetProviderName.vi"("ClassWriterNative in"=w261, "error in (no error)"=w258) -> ("ProviderName"=w241:string, "error out"=w248:errorcluster)  [unwired: 13 in, 3 out]
            n125 = case shown="\"EndevoGOOP400\"" w241 {
              tunnel: ["OpenG Reference Object" ("Child Tag") "Root Object" ("Child Tag") "LabVIEW Object" ("Child Tag") "LabVIEW Object" ("Child Tag")] -> w251
              tunnel: [TRUE TRUE _ _] -> w249
              frame "OpenG100" {
              }
              frame "OpenG200" {
              }
              frame "EndevoGOOP400" {
              }
              frame Default {
              }
            }
            n126 = Unbundle By Name(w253) -> ("DeriveFromClass"=w246:path)
            n127 = local read "ParentClassFilter"() -> (w235:string)
            n128 = invoke class="Tree (strict)" method="Edit Tree Items.Delete"(reference=w262, error in=w248) -> (reference out=w260:refnum<vi>, error out=w259:errorcluster)  [unwired: 3 in, 3 out]
            n129 = Build Array("Select this to make a base class" ("Child Tag")) -> (w256:string[])
            n130 = Equal?(x="Parent class name filter", y=w235) -> (x = y?=w236:bool)
            n131 = invoke class="Tree (strict)" method="Edit Tree Items.Add Item to End"(reference=w260, error in=w259, "Left Cell"=w251, "Child Text"=w256, "Child Tag"=w251) -> (reference out=w254:refnum<vi>)  [unwired: 3 in, 7 out]
            n132 = Select(t="", s=w236, f=w235) -> (s? t:f=w234:string)
            n133 = call <resource>:"GDSProject_GetAllClasses.vi"("AnyProjectItemRefnum"=w240, "TreeControlRef"=w254, "ClassProviderName"=w241, "RootParentTag"=w251, "error In"=w248, "Interfaces(False)"=FALSE, "ClassFilter"=w234) -> ("ClassPaths"=w247:path[], "ClassTags"=w244:string[], "error out"=w238:errorcluster)  [unwired: 10 in]
            n134 = Search 1D Array(1D array=w247, element=w246) -> (index of element=w245:i32)  [unwired: 1 in]
            n135 = Index Array(array=w244, index=w245) -> (element=w243:string)
            n136 = Empty String/Path?(string/path=w243) -> (empty?=w252:bool)
            n137 = Select(t=w251, s=w252, f=w243) -> (s? t:f=w250:string)
            n138 = Bundle By Name(cluster=w253, "BaseObjectTag"=w251, "OpenG"=w249, "ClassPaths"=w247, "ClassTags"=w244) -> (w255:T13)
            n139 = stacked-sequence {
              tunnel: w250 -> [w269]
              tunnel: w238 -> [_]
              frame #0 {
                n140 = local write "_SelectParentClass"(w269) -> ()
                n141 = Bundle By Name(cluster=T16 {"Node"="", "Column"=0} ("Top Left Visible Cell"), "Node"=w269) -> (w270:T16)
                n142 = property on="_SelectParentClass" class="Tree (strict)"("TopLeft"=w270) -> ()  [unwired: 2 in, 2 out]
              }
            }
          }
          frame "CreateInterfaceList" {
            n143 = call <resource>:"GetInterfacesInProject.vi"("error in"=w272, "Project/ProjectItem"=w283) -> ("error out"=w279:errorcluster, "InterfaceInfo"=w282:T11[])  [unwired: 8 in]
            n144 = for {
              tunnel: w282 -> [w295] mode=indexing
              tunnel: [w294] -> w281 mode=indexing
              n145 = Unbundle By Name(w295) -> ("IconPath"=w294:path)
            }
            n146 = call "Remove Duplicates From 1D Array.vim"("array"=w281) -> ("array with duplicates removed"=w280:path[])  [unwired: 10 in]
            n147 = for {
              tunnel: w280 -> [w293] mode=indexing
              shift-right: [w287] -> w278
              shift-left: w279 -> [w287]
              tunnel: [w286] -> w277 mode=indexing
              n148 = call <vilib>:"Read PNG File.vi"("path to PNG file"=w293) -> ("image data"=w292:T17)  [unwired: 8 in, 2 out]
              n149 = call <vilib>:"Unflatten Pixmap.vi"("image data"=w292) -> ("24-bit pixmap"=w291:u32[][])  [unwired: 4 in, 6 out]
              n150 = Array Subset(array=w291, index (col)=4 ("index"), length (col)=16 ("length")) -> (w288:u32[][])  [unwired: 2 in]
              n151 = call <vilib>:"Flatten Pixmap.vi"("24-bit pixmap"=w288) -> ("image data"=w286:T17)  [unwired: 10 in]
            }
            n152 = Bundle By Name(cluster=w284, "InterfaceInfo"=w282, "InterfaceIcons"=w280) -> (w285:T13)
            n153 = Build Array (concatenate)(T17 {"image type"=0, "image depth"=0, "image"=[], "mask"=[], "colors"=[], "Rectangle"={"left"=0, "top"=0, "right"=0, "bottom"=0}} ("image data"), w277) -> (w274:T17[])
            n154 = invoke on="_SelectInterfaceClass" class="MCListbox (strict)" method="Custom Item Symbols.Set Symbol Array"(error in=w278, "symbols"=w274) -> (error out=w276:errorcluster)  [unwired: 2 in, 3 out]
          }
          frame "UpdateInterfaceList" {
            n155 = local read "InterfaceFilter"() -> (w319:string)
            n156 = Unbundle By Name(w324) -> ("StartInterfacePath"=w309:path, "InterfaceIcons"=w322:path[], "InterfaceInfo"=w323:T11[])
            n157 = call <vilib>:"Trim Whitespace.vi"("string"=w319) -> ("trimmed string"=w314:string)  [unwired: 1 in]
            n158 = Empty String/Path?(string/path=w314) -> (empty?=w317:bool)
            n159 = Equal?(x=w314, y="Interface name filter" ("InterfaceFilter")) -> (x = y?=w316:bool)
            n160 = To Lower Case(string=w314) -> (all lower case string=w312:string)
            n161 = Compound Arithmetic op=OR(w317, w316) -> (w315:bool)
            n162 = for {
              tunnel: [w346] -> w321 mode=indexing if=w336
              tunnel: w323 -> [w345] mode=indexing
              tunnel: w322 -> [w342]
              tunnel: [w341] -> w311 mode=indexing if=w336
              tunnel: w315 -> [w340]
              tunnel: w312 -> [w338]
              tunnel: [w337] -> w299 mode=indexing if=w336
              n163 = Unbundle By Name(w345) -> ("Path"=w337:path, "IconPath"=w343:path, "Name(Short if no Conflicts)"=w339:string, "Description"=w335:string, "ParentInterfaceNames(Short if no Conflitcs)"=w344:string[])
              n164 = case shown="False" w340 {
                tunnel: [w352 TRUE] -> w336
                tunnel: w339 -> [w355 _]
                tunnel: w338 -> [w354 _]
                frame False {
                  n165 = To Lower Case(string=w355) -> (all lower case string=w351:string)
                  n166 = Match Pattern(string=w351, regular expression=w354) -> (offset past match=w353:i32)  [unwired: 1 in, 3 out]
                  n167 = Greater Or Equal To 0?(x=w353) -> (x >= 0?=w352:bool)
                }
                frame True {
                }
              }
              n168 = Array To Spreadsheet String(delimiter (Tab)=",", array=w344, 3:"%s" ("format string")) -> (spreadsheet string=w348:string)
              n169 = call <vilib>:"Trim Whitespace.vi"("string"=w348) -> ("trimmed string"=w347:string)  [unwired: 1 in]
              n170 = call <vilib>:"Trim Whitespace.vi"("string"=w335) -> ("trimmed string"=w334:string)  [unwired: 1 in]
              n171 = Search 1D Array(1D array=w342, element=w343) -> (index of element=w341:i32)  [unwired: 1 in]
              n172 = call <vilib>:"Search and Replace Pattern.vi"("string"=w334, "regular expression (\"\")"="[\\n\\r]+" ("regular expression (\"\")"), "replace string (\"\")"=" " ("replace string (\"\")"), "replace all? (F)"=TRUE) -> ("result string"=w330:string)  [unwired: 1 in, 1 out]
              n173 = Build Array(w339, w347, w330) -> (w346:string[])
            }
            n174 = Search 1D Array(1D array=w299, element=w309) -> (index of element=w306:i32)  [unwired: 1 in]
            n175 = Greater Or Equal?(x=w306, y=4) -> (x >= y?=w304:bool)
            n176 = case shown="0, Default" w306 {
              selector: w306 -> [w328 _]
              tunnel: [w327 i32[] [] ("_SelectInterfaceClass")] -> w298
              frame 0, Default {
                n177 = Build Array(w328) -> (w327:i32[])
              }
              frame -1 {
              }
            }
            n178 = Subtract(x=w306, y=2) -> (x-y=w303:i32)
            n179 = Select(t=w303, s=w304, f=0) -> (s? t:f=w302:i32)
            n180 = Bundle By Name(cluster=T18 {"Row"=0, "Column"=0} ("Top Left Visible Cell"), "Row"=w302) -> (w307:T18)
            n181 = property on="_SelectInterfaceClass" class="MCListbox (strict)"("ItemNames"=w321, "Value"=w298, "TopLeft"=w307) -> (error out=w320:errorcluster)  [unwired: 2 in, 1 out]
            n182 = Bundle By Name(cluster=w324, "InterfacesInList"=w299) -> (w300:T13)
            n183 = Increment(x=w311) -> (x+1=w310:i32[])
            n184 = Empty Array?(array=w298) -> (empty?=w297:bool)
            n185 = call <resource>:"GDSControl_Disable.vi"("Disasble(True)"=w297) -> ("Enable Property"=w296:T19)  [unwired: 10 in]
            n186 = property on="CreateInterfaceMethods" class="Enum (strict)"("DisabledEnum"=w296) -> ()  [unwired: 2 in, 2 out]
            n187 = property on="_SelectInterfaceClass" class="MCListbox (strict)"(error in=w320, "ItemSyms"=w310) -> ()  [unwired: 1 in, 2 out]
          }
          frame "UpdateClassProviderList" {
            n188 = Unbundle By Name(w366) -> ("Derived"=w371:bool)
            n189 = call-dynamic "GetProviderName.vi"("ClassWriterNative in"=w367) -> ("ProviderName"=w359:string)  [unwired: 14 in, 4 out]
            n190 = call <resource>:"GOOP_CurrentProviderClass_Memory.vi"() -> ("AllClassProviders(OriginalNames)"=w357:string[], "AllClassProviders(TranslatedNames)"=w361:string[])  [unwired: 13 in, 5 out]
            n191 = Search 1D Array(1D array=w357, element=w359) -> (index of element=w363:i32)  [unwired: 1 in]
            n192 = case shown="0, Default" w363 {
              selector: w363 -> [w376 _]
              tunnel: [w376 w379] -> w362
              tunnel: w361 -> [w375 _]
              tunnel: [w375 w378] -> w360
              tunnel: w359 -> [_ w380]
              tunnel: [w374 w377] -> w358
              tunnel: w357 -> [w374 _]
              frame 0, Default {
              }
              frame -1 {
                n193 = call <resource>:"GOOP_CurrentProviderClass_Memory.vi"("IgnoreFilter(False)"=TRUE) -> ("AllClassProviders(OriginalNames)"=w377:string[], "AllClassProviders(TranslatedNames)"=w378:string[])  [unwired: 12 in, 5 out]
                n194 = Search 1D Array(1D array=w377, element=w380) -> (index of element=w379:i32)  [unwired: 1 in]
              }
            }
            n195 = Select(t=T19."Disabled and Grayed Out" ("Disabled"), s=w371, f=T19."Enabled" ("Disabled")) -> (s? t:f=w370:T19)
            n196 = Bundle By Name(cluster=w366, "ChangeProviderTo"="", "Providers"=w358) -> (w365:T13)
            n197 = property on="_CurrentClassProvider" class="Ring (strict)"("Strings []"=w360, "Value"=w362, "DisabledEnum"=w370) -> ()  [unwired: 2 in, 2 out]
          }
          frame "GetTemplates" {
            n198 = Unbundle By Name(w405) -> ("InitDerived"=w410:bool, "Derived"=w417:bool, "OpenG"=w411:bool, "DeriveFromClassRef"=w384:refnum<vi>)
            n199 = call-dynamic "GetClassTemplates.vi"("ClassWriterNative in"=w383, "DerivedFromThisClass(if any)"=w384, "error in (no error)"=w418) -> ("ClassWriterNative out"=w385:refnum<class "ClassWriterNative.lvclass">, "Templates(Matching Connector Pane Settings)"=w387:T10[], "AllTemplateNames(FolderNames)"=w386:string[], "error out"=w420:errorcluster)  [unwired: 13 in]
            n200 = call <resource>:"GOOP_AddCustomClassTemplates.vi"("DerivedFromThisClass(if any)"=w384, "BuildInTemplates"=w386, "TemplateIdNamesIn"=w387, "ClassWriter in"=w385) -> ("TemplateIdNamesOut"=w388:T10[])  [unwired: 7 in]
            n201 = call-dynamic "GetProviderName.vi"("ClassWriterNative in"=w383) -> ("ShortName(Could be used in for INI Sections)"=w382:string)  [unwired: 14 in, 4 out]
            n202 = Unbundle By Name(w405) -> ("ClassProviderName"=w404:string)
            n203 = case shown="True" w417 {
              tunnel: w420 -> [w462 w467]
              tunnel: w384 -> [_ w463]
              tunnel: [w462 w466] -> w391
              tunnel: [_ w464] -> w414
              frame False {
              }
              frame True {
                n204 = call <resource>:"GDSLvClass_ReadClassType.vi"("Class Refnum In"=w463, "error in (no error)"=w467) -> ("ClassSettings"=w468:T21, "error out"=w466:errorcluster)  [unwired: 15 in, 1 out]
                n205 = Unbundle By Name(w468) -> ("ClassTemplateUsed"=w465:string)
                n206 = call <resource>:"GOOP_ClassTemplateSplit.vi"("ClassItemRefIn"=w463, "FullClassTemplate"=w465) -> ("StandardTemplate"=w464:string)  [unwired: 12 in, 1 out]
              }
            }
            n207 = case shown="False" w411 {
              tunnel: w388 -> [w429 w456]
              tunnel: w417 -> [w427 _]
              tunnel: [w426 w456] -> w395
              tunnel: w414 -> [w425 _]
              frame False {
                n208 = for {
                  N: 2 -> [_]
                  tunnel: w429 -> [w439]
                  tunnel: T10[] [] -> [w438]
                  tunnel: w427 -> [w432]
                  tunnel: [w436] -> w426
                  tunnel: w425 -> [w437]
                  i -> [w434]
                  stop <- w430 continue-if-true
                  n209 = Equal To 0?(x=w434) -> (x = 0?=w433:bool)
                  n210 = And(x=w432, y=w433) -> (x .and. y?=w431:bool)
                  n211 = for {
                    tunnel: w439 -> [w449] mode=indexing
                    shift-right: [w451] -> w436
                    shift-left: w438 -> [w450]
                    tunnel: w437 -> [w447]
                    tunnel: w431 -> [w443]
                    n212 = Unbundle By Name(w449) -> ("OnlySubClassTemplate"=w444:bool, "CanDeriveFromTheseTemplateIDs"=w448:string[])
                    n213 = Search 1D Array(1D array=w448, element=w447) -> (index of element=w441:i32)  [unwired: 1 in]
                    n214 = Compound Arithmetic op=AND(invert w443, invert w444) -> (w445:bool)
                    n215 = Greater Or Equal To 0?(x=w441) -> (x >= 0?=w442:bool)
                    n216 = Compound Arithmetic op=AND(w443, w442) -> (w440:bool)
                    n217 = Or(x=w445, y=w440) -> (x .or. y?=w446:bool)
                    n218 = case shown="False" w446 {
                      tunnel: w450 -> [w452 w455]
                      tunnel: [w452 w453] -> w451
                      tunnel: w449 -> [_ w454]
                      frame False {
                      }
                      frame True {
                        n219 = Build Array (concatenate)(w455, w454) -> (w453:T10[])
                      }
                    }
                  }
                  n220 = Array Size(array=w436) -> (size(s)=w435:i32)
                  n221 = Equal To 0?(x=w435) -> (x = 0?=w430:bool)
                }
              }
              frame True {
              }
            }
            n222 = Index Array(array=w395) -> (element=w394:T10)  [unwired: 1 in]
            n223 = Unbundle By Name(w394) -> ("TemplateIdName"=w393:string)
            n224 = call <resource>:"BaseProvider_ActorFramework_FindTemplates.vi"("MainClassemplateID"=w393, "FilterOnProviders"=w404, "DeriveFromClassRef"=w384) -> ("Array"=w407:T10[])  [unwired: 7 in, 1 out]
            n225 = Build Array (concatenate)(w407, w395) -> (w406:T10[])
            n226 = Array Size(array=w406) -> (size(s)=w416:i32)
            n227 = call <resource>:"DialogCreateClass_FilterAndOrderClassTemplates.vi"("ProviderShortName"=w382, "error in (no error)"=w391, "AllTemplatesForThisProvider/InheritanceType(Base/Sub)"=w406) -> ("error out"=w390:errorcluster, "NewOrderIndex"=w389:i32[], "FilteredTemplates"=w392:T10[])  [unwired: 6 in]
            n228 = for {
              tunnel: w392 -> [w461] mode=indexing
              tunnel: [w460] -> w419 mode=indexing
              tunnel: [w459] -> w415 mode=indexing
              tunnel: [w458] -> w409 mode=indexing
              tunnel: [w457] -> w403 mode=indexing
              n229 = Unbundle(w461) -> ("TemplateIdName"=w459:string, "TemplateUserDialogName"=w460:string, "ClassSuffix"=w458:string, "LvLibTemplate"=w457:bool)  [unwired: 4 out]
            }
            n230 = Bundle By Name(cluster=w405, "Templates"=w406, "ClassTemplateIndex"=w389) -> (w421:T13)
            n231 = Search 1D Array(1D array=w415, element=w414) -> (index of element=w413:i32)  [unwired: 1 in]
            n232 = property on="_ClassType" class="LstBox (strict)"("Value"=-1 ("_ClassType")) -> (error out=w396:errorcluster)  [unwired: 2 in, 1 out]
            n233 = Max & Min(x=w413, y=0 ("Class Type")) -> (max(x,y)=w402:i32)  [unwired: 1 out]
            n234 = case shown="0" w416 {
              tunnel: ["ChangeTheStartPath?" w472] -> w422
              tunnel: w410 -> [_ w470]
              frame Default {
              }
              frame 0 {
                n235 = case shown="False" w470 {
                  tunnel: ["ChangeTheStartPath?" "Exit"] -> w472
                  frame False {
                  }
                  frame True {
                  }
                }
                n236 = One Button Dialog(message="This class provider don't\nhave a sub class template\nto use when deriving for\nthe selected class.") -> ()  [unwired: 1 in, 1 out]
              }
            }
            n237 = Index Array(array=w409, index=w402) -> (element=w408:string)
            n238 = Index Array(array=w403, index=w402) -> (element=w401:bool)
            n239 = property on="_ClassType" class="LstBox (strict)"(error in=w396, "Item Names"=w419, "Val(Sgnl)"=w402) -> ()  [unwired: 1 in, 2 out]
            n240 = case shown="Default" w408 {
              selector: w408 -> [_ w423]
              frame "" {
              }
              frame Default {
                n241 = property on="_ClassFolderSuffix" class="Str"("Val(Sgnl)"=w423) -> ()  [unwired: 2 in, 2 out]
              }
            }
            n242 = Select(t="Library folder (The lvlib file will be saved in this directory)", s=w401, f=w398) -> (s? t:f=w399:string)
            n243 = property on="_ClassFolder" class="Path"("Caption.Text"=w399) -> ()  [unwired: 2 in, 2 out]
          }
          frame "ChangeTheStartPath?" {
            n244 = Unbundle By Name(w483) -> ("StartFolder"=w477:path, "DeriveFromClassRef"=w481:refnum<vi>)
            n245 = Not A Number/Path/Refnum?(number/path/refnum=w481) -> (NaN/Path/Refnum?=w478:bool)
            n246 = case shown="False" w478 {
              tunnel: w481 -> [w489 _]
              tunnel: [w490 _] -> w480
              tunnel: [w493 _] -> w476
              frame False {
                w487 = "Actor Framework.lvlib:Actor.lvclass" ("y")
                n247 = property class="LVClassLibrary"(reference=w489) -> ("Parent"=w500:refnum<vi>)  [unwired: 1 in, 2 out]
                n248 = call <resource>:"GDSLvClass_GetRootBaseClass.vi"("ViRef/Path,LvClassRef/Path"=w489, "Don'tOpenReference"=FALSE, "LimitToSpecificProviderTypeOfSameType(True)"=FALSE) -> ("RootBaseClassRef"=w501:refnum<vi>)  [unwired: 10 in, 6 out]
                n249 = property class="LVClassLibrary"(reference=w501) -> (reference out=w502:refnum<vi>, "QualifiedName"=w504:string)  [unwired: 1 in, 1 out]
                n250 = property class="LVClassLibrary"(reference=w489) -> ("QualifiedName"=w488:string)  [unwired: 1 in, 2 out]
                n251 = property class="ProjectItem"(reference=w500) -> (reference out=w496:refnum<vi>, error out=w497:errorcluster, "Type String"=w499:string, "Path"=w495:path)  [unwired: 1 in]
                n252 = Equal?(x=w489, y=w502) -> (x = y?=w503:bool)
                n253 = Equal?(x=w504, y=w487) -> (x = y?=w492:bool)
                n254 = Not Equal?(x=w487, y=w488) -> (x != y?=w486:bool)
                n255 = case shown="False" w503 {
                  tunnel: w502 -> [w507 _]
                  frame False {
                    n256 = Close Reference(reference=w507) -> ()  [unwired: 1 in, 1 out]
                  }
                  frame True {
                  }
                }
                n257 = Strip Path(path=w495) -> (stripped path=w494:path)  [unwired: 1 out]
                n258 = Equal?(x=w499, y="Library") -> (x = y?=w491:bool)
                n259 = Close Reference(reference=w496, error in (no error)=w497) -> ()  [unwired: 1 out]
                n260 = Strip Path(path=w494) -> (stripped path=w493:path)  [unwired: 1 out]
                n261 = Compound Arithmetic op=AND(w492, w486, w491) -> (w490:bool)
              }
              frame True {
              }
            }
            n262 = local read "_ClassName"() -> (w475:string)
            n263 = Select(t=w476, s=w480, f=w477) -> (s? t:f=w482:path)
            n264 = case shown="Default" w475 {
              selector: w475 -> [w485 _]
              frame Default {
                n265 = property on="_ClassName" class="Str"("Val(Sgnl)"=w485) -> ()  [unwired: 2 in, 2 out]
              }
              frame "" {
              }
            }
            n266 = property on="_ClassFolder" class="Path"("StartPath"=w482, "Value"=w482) -> ()  [unwired: 2 in, 2 out]
          }
          frame "GetClassInfo" {
          }
          frame "", "Idle" {
            w512 = i16 386  # Width of Design Pattern Pane
            n267 = local read "_ClassFolder"() -> (w528:path)
            n268 = Unbundle By Name(w518) -> ("Templates"=w513:T10[], "ClassTemplateIndex"=w516:i32[])
            n269 = local read "_ClassName"() -> (w531:string)
            n270 = local read "_ClassType"() -> (w530:i32)
            n271 = local read "_ClassType"() -> (w515:i32)
            n272 = List Folder(path=w528, pattern="*.lvclass") -> (filenames=w526:string[])  [unwired: 2 in, 3 out]
            n273 = Index Array(array=w516, index=w515) -> (element=w514:i32)
            n274 = Empty String/Path?(string/path=w528) -> (empty?=w533:bool)
            n275 = Array Size(array=w526) -> (size(s)=w525:i32)
            n276 = Empty String/Path?(string/path=w531) -> (empty?=w532:bool)
            n277 = Less Than 0?(x=w530) -> (x < 0?=w529:bool)
            n278 = Greater Than 0?(x=w525) -> (x > 0?=w524:bool)
            "DupPath" <- w524
            n279 = Index Array(array=w513, index=w514) -> (element=w519:T10)
            n280 = Compound Arithmetic op=OR(w524, w533, w532, w529) -> (w534:bool)
            n281 = Select(t=u8 2, s=w534, f=u8 0 ("Disabled")) -> (s? t:f=w537:u8)
            n282 = Unbundle By Name(w519) -> ("LvLibTemplate"=w517:bool)
            n283 = property on="_CreateClass" class="Bool"("Disabled"=w537) -> ()  [unwired: 2 in, 2 out]
            n284 = event shown="[9] \"ModifyTemplates\": Value Change" {
              selector: _ -> [_ _ _ _ _ _ _ _ _ _ _ _ _ _ _ _ _ _ _ _ _ _ _ _]
              dyn-events: _ -> [_ _ _ _ _ _ _ _ _ _ _ _ _ _ _ _ _ _ _ _ _ _ _ _]
              timeout: _ -> [_ _ _ _ _ _ _ _ _ _ _ _ _ _ _ _ _ _ _ _ _ _ _ _]
              tunnel: ["Exit" _ "Exit" "Idle" "Exit" "GetClassTemplateToUse" "Idle" w635 "Idle" w670 w680 "GetTemplates" "Idle" "Idle" "Idle" "Idle" w839 "UpdateInterfaceList" "CreateClassTree" _ "Idle" "Idle" "Idle" "Idle"] -> w539
              tunnel: [TRUE _ w595 _ FALSE ("Cancel") _ _ _ _ _ w678 _ _ _ _ _ _ _ _ _ _ _ _ _] -> w540
              tunnel: w518 -> [_ w549 _ _ w606 _ _ w631 w655 _ _ _ w701 w713 w754 _ w844 _ _ w871 _ _ _ _]
              tunnel: w523 -> [_ _ _ _ _ _ _ _ _ _ _ _ _ _ _ _ _ _ _ _ _ _ _ _]
              tunnel: w518 -> [w543 w560 w594 w597 w611 w613 w617 w634 w657 w677 w683 w696 w702 w716 w756 w804 w841 w863 w865 w870 w877 w885 w900 w910]
              tunnel: [w542 w556 w594 w597 w610 w615 w617 w633 w657 w674 w682 w696 w702 w716 w756 w804 w840 w863 w865 w869 w877 w885 w900 w910] -> w522
              tunnel: w521 -> [_ _ _ _ _ _ _ _ _ _ _ _ _ _ _ _ _ _ _ _ _ _ _ _]
              tunnel: w520 -> [_ _ _ _ _ _ _ _ w649 _ _ _ _ _ _ _ _ _ _ _ _ _ _ _]
              tunnel: w517 -> [_ _ _ _ _ _ _ _ _ _ _ _ _ _ _ w803 _ _ _ _ _ _ w892 _]
              tunnel: w513 -> [_ _ _ _ _ _ _ _ _ w676 _ _ _ _ _ _ _ _ _ _ _ _ _ _]
              tunnel: w512 -> [_ w547 _ _ _ _ _ w623 _ _ _ _ _ _ _ _ _ _ _ _ _ _ _ _]
              tunnel: [_ _ _ _ _ w613 _ _ _ _ _ _ _ _ _ _ _ _ _ _ _ _ _ _] -> _
              tunnel: w511 -> [_ _ _ _ _ _ _ _ _ w675 _ _ _ _ _ _ _ _ _ _ _ _ _ _]
              event "_Cancel": Value Change {
                n285 = event-data() -> ()  [unwired: 1 in, 2 out]
                n286 = Bundle By Name(cluster=w543, "LastProvderValues"=T20 {"_ClassName"="", "_ClassFolder"=path "", "_ClassDescription"="", "seconds since 1Jan1904"=timestamp(0 s since 1904-01-01)}) -> (w542:T13)
              }
              event Panel Resize {
                n287 = event-data() -> ("OldBnds"=w557:T9, "NewBnds"=w551:T9)  [unwired: 1 in]
                n288 = Unbundle By Name(w549) -> ("DesignPatternsVisible"=w548:bool)
                n289 = Unbundle By Name(w549) -> ("StartBnds"=w550:T9, "OldBnds"=w558:T9, "BondsChanged"=w554:bool)
                n290 = property class="VI"() -> ("FP.State"=w552:T26)  [unwired: 2 in, 2 out]
                n291 = Equal?(x=w557, y=w551) -> (x = y?=w559:bool)
                n292 = case shown="\"Standard\", Default" w552 {
                  tunnel: w559 -> [_ w576]
                  tunnel: w558 -> [_ w575]
                  tunnel: w557 -> [w562 w574]
                  tunnel: [FALSE w573] -> w555
                  tunnel: w554 -> [_ w572]
                  tunnel: [w562 w571] -> w553
                  tunnel: w551 -> [w564 _]
                  tunnel: w550 -> [w563 w570]
                  tunnel: w548 -> [_ w569]
                  tunnel: w547 -> [_ w568]
                  frame "Maximized" {
                    n293 = Unbundle By Name(w564) -> ("Top"=w565:i16, "Bottom"=w566:i16)
                    n294 = Bundle By Name(cluster=w563, "Top"=w565, "Bottom"=w566) -> (w567:T9)
                    n295 = property class="VI"("Front Panel.PanelBounds"=w567) -> ()  [unwired: 2 in, 2 out]
                  }
                  frame "Standard", Default {
                    n296 = case shown="True" w576 {
                      tunnel: w574 -> [w578 w589]
                      tunnel: [w579 w589] -> w571
                      tunnel: w575 -> [w580 _]
                      tunnel: [TRUE FALSE] -> w573
                      tunnel: w572 -> [w577 _]
                      tunnel: w570 -> [_ w588]
                      tunnel: w569 -> [_ w587]
                      tunnel: w568 -> [_ w583]
                      frame False {
                        n297 = Select(t=w580, s=w577, f=w578) -> (s? t:f=w579:T9)
                      }
                      frame True {
                        n298 = Unbundle By Name(w589) -> ("Top"=w593:i16, "Bottom"=w592:i16)
                        n299 = Unbundle By Name(w588) -> ("Right"=w585:i16)
                        n300 = Select(t=w583, s=w587, f=i16 0) -> (s? t:f=w586:i16)
                        n301 = Add(x=w585, y=w586) -> (x+y=w584:i16)
                        n302 = Bundle By Name(cluster=w588, "Top"=w593, "Bottom"=w592, "Right"=w584) -> (w591:T9)
                        n303 = property class="VI"("Front Panel.PanelBounds"=w591) -> ()  [unwired: 2 in, 2 out]
                      }
                    }
                  }
                }
                n304 = Bundle By Name(cluster=w560, "OldBnds"=w553, "BondsChanged"=w555) -> (w556:T13)
              }
              event Panel Close? {
                w595 = TRUE
                n305 = event-data() -> ()  [unwired: 1 in, 2 out]
                n306 = event-data("Discard?"=w595) -> ()  [unwired: 1 in, 1 out]
              }
              event "Help": Value Change {
                n307 = event-data() -> ()  [unwired: 1 in, 2 out]
                n308 = call <resource>:"GOOP_HelpMain.vi"() -> ()  [unwired: 12 in]
              }
              event "_CurrentClassProvider": Value Change {
                n309 = event-data() -> ()  [unwired: 1 in, 2 out]
                n310 = Unbundle By Name(w606) -> ("Providers"=w605:string[], "LastProvderValues"=w600:T27)
                n311 = local read "_ClassName"() -> (w604:string)
                n312 = local read "_ClassFolder"() -> (w603:path)
                n313 = local read "_ClassDescription"() -> (w602:string)
                n314 = Get Date/Time In Seconds() -> (seconds since 1Jan1904=w601:timestamp)
                n315 = Bundle(cluster=w600, "_ClassName"=w604, "_ClassFolder"=w603, "_ClassDescription"=w602, "Created"=w601) -> (w599:T27)
                n316 = Index Array(array=w605, index="_CurrentClassProvider") -> (element=w608:string)
                n317 = Bundle By Name(cluster=w611, "ChangeProviderTo"=w608, "LastProvderValues"=w599) -> (w610:T13)
              }
              event "_CreateClass": Value Change {
                n318 = event-data() -> ()  [unwired: 1 in, 2 out]
                n319 = Bundle By Name(cluster=w613, "LastProvderValues"=T20 {"_ClassName"="", "_ClassFolder"=path "", "_ClassDescription"="", "seconds since 1Jan1904"=timestamp(0 s since 1904-01-01)}) -> (w615:T13)
              }
              event "_ClassDescription": Value Change {
                n320 = event-data() -> ()  [unwired: 1 in, 2 out]
              }
              event "AddDesignPattern": Value Change {
                n321 = event-data() -> ()  [unwired: 1 in, 2 out]
                n322 = Unbundle By Name(w631) -> ("DPDescriptions"=w622:string[])
                n323 = Unbundle By Name(w631) -> ("DesignPatternsVisible"=w626:bool)
                n324 = Array Size(array=w622) -> (size(s)=w621:i32)
                n325 = Not(x=w626) -> (.not. x?=w632:bool)
                n326 = Initialize Array(37, w621) -> (w619:i32[])
                n327 = property on="DesignPatternList" class="LstBox (strict)"("Item Symbols"=w619) -> ()  [unwired: 2 in, 2 out]
                n328 = property class="VI"() -> ("Front Panel.PanelBounds"=w629:T9)  [unwired: 2 in, 2 out]
                n329 = case shown="True" w632 {
                  tunnel: ["Idle" "GetDesignPatterns"] -> w635
                  frame False {
                  }
                  frame True {
                  }
                }
                n330 = Negate(x=w623) -> (-x=w625:i16)
                n331 = Unbundle By Name(w629) -> ("Right"=w630:i16)
                n332 = Select(t=w625, s=w626, f=w623) -> (s? t:f=w624:i16)
                n333 = Add(x=w630, y=w624) -> (x+y=w627:i16)
                n334 = Bundle By Name(cluster=w634, "DesignPatternsVisible"=w632) -> (w633:T13)
                n335 = Bundle By Name(cluster=w629, "Right"=w627) -> (w628:T9)
                n336 = property class="VI"("Front Panel.PanelBounds"=w628) -> ()  [unwired: 2 in, 2 out]
              }
              event "_ClassType": Value Change {
                n337 = event-data() -> ()  [unwired: 1 in, 2 out]
                n338 = Unbundle By Name(w655) -> ("Templates"=w654:T10[], "ClassFolderSuffix"=w651:string, "LLB_Allowed"=w642:bool, "ClassTemplateIndex"=w640:i32[])
                n339 = property on="_ClassFolderSuffix" class="Str"() -> (error out=w647:errorcluster, "Value"=w644:string)  [unwired: 2 in, 1 out]
                n340 = Index Array(array=w640, index="_ClassType") -> (element=w638:i32)
                n341 = Index Array(array=w654, index=w638) -> (element=w653:T10)
                n342 = Unbundle By Name(w653) -> ("ClassSuffix"=w652:string, "LvLibTemplate"=w643:bool)
                n343 = case shown="\"\"" w652 {
                  selector: w652 -> [_ w668]
                  tunnel: w651 -> [w667 _]
                  tunnel: [w667 w668] -> w646
                  frame "" {
                  }
                  frame Default {
                  }
                }
                n344 = Not Equal?(x=w644, y=w646) -> (x != y?=w645:bool)
                n345 = case shown="False" w645 {
                  tunnel: w644 -> [_ w662]
                  frame False {
                  }
                  frame True {
                    n346 = local read "_ClassFolder"() -> (w661:path)
                    n347 = Concatenate Strings(w662, "$" ("string")) -> (w665:string)
                    n348 = Strip Path(path=w661) -> (stripped path=w663:path, name=w666:string)
                    n349 = Match Pattern(string=w666, regular expression=w665) -> (before substring=w660:string)  [unwired: 1 in, 3 out]
                    n350 = Build Path(base path=w663, name or relative path=w660) -> (appended path=w659:path)
                    n351 = local write "_ClassFolder"(w659) -> ()
                  }
                }
                n352 = Select(t="Library folder (The lvlib file will be saved in this directory)", s=w643, f=w649) -> (s? t:f=w650:string)
                n353 = Compound Arithmetic op=AND(invert w643, w642) -> (w641:bool)
                n354 = property on="_ClassFolder" class="Path"("Caption.Text"=w650) -> ()  [unwired: 2 in, 2 out]
                n355 = property on="_UseLLB" class="Bool (strict)"("Visible"=w641) -> ()  [unwired: 2 in, 2 out]
                n356 = property on="_ClassFolderSuffix" class="Str"(error in=w647, "Val(Sgnl)"=w646) -> ()  [unwired: 1 in, 2 out]
                n357 = case shown="False" w641 {
                  frame False {
                    n358 = local write "_UseLLB"(FALSE ("_UseLLB")) -> ()
                  }
                  frame True {
                  }
                }
              }
              event "ModifyTemplates": Value Change {
                n359 = event-data() -> ()  [unwired: 1 in, 6 out]
                n360 = call <resource>:"DialogCreateClass_HandleTemplatesDialog.vi"("AllTemplatesForThisProvider/InheritanceType(Base/Sub)"=w676, "ClassWriter in"=w675) -> ("TemplatesOut"=w673:T10[], "RefreshClassTemplates"=w672:bool)  [unwired: 7 in, 1 out]
                n361 = Select(t="GetTemplates", s=w672, f="UpdateTemplates") -> (s? t:f=w670:string)
                n362 = Bundle By Name(cluster=w677, "Templates"=w673) -> (w674:T13)
              }
              event "ModifyProviders": Value Change {
                n363 = event-data() -> ()  [unwired: 1 in, 6 out]
                n364 = call <resource>:"GOOP_ProviderClasses_SortingDialog.vi"() -> ("Cancelled"=w679:bool, "FirstProvider"=w681:string)  [unwired: 9 in, 1 out]
                n365 = case shown="False" w679 {
                  tunnel: w683 -> [w688 w689]
                  tunnel: [w687 w689] -> w682
                  tunnel: w681 -> [w686 _]
                  tunnel: ["Exit" _] -> w680
                  tunnel: [FALSE ("Cancel") _] -> w678
                  frame False {
                    n366 = Bundle By Name(cluster=w688, "ChangeProviderTo"=w686) -> (w687:T13)
                  }
                  frame True {
                  }
                }
              }
              event Value Change {
                n367 = event-data() -> ()  [unwired: 1 in, 6 out]
                n368 = call <resource>:"BaseProvider_ConfigurationMemory.vi"() -> ("WireConfigurationOut"=w692:T28, "IconOut"=w691:string, "error out"=w695:errorcluster)  [unwired: 13 in, 4 out]
                n369 = call <resource>:"BaseProvider_ConfigurationMemory.vi"("WireConfiguration"=w692, "Icon"=w691, "error in (no error)"=w695, "Action"=enum16{"Read", "Load", "Save", "Set"}."Save", "PatternIn"="ConnectorPanePattern") -> ()  [unwired: 8 in, 7 out]
              }
              event "DesignPatternList": Value Change {
                n370 = event-data() -> ()  [unwired: 1 in, 2 out]
                n371 = Unbundle By Name(w701) -> ("DPDescriptions"=w700:string[])
                n372 = Index Array(array=w700, index="DesignPatternList") -> (element=→"DesignPatternDescription":string)
              }
              event "DesignPatternList": Double Click {
                n373 = event-data() -> ("Row"=w704:i32)  [unwired: 1 in]
                n374 = Unbundle By Name(w713) -> ("DpDependencies"=w712:cluster{"DependenciesID":string[]}[], "DPs"=w705:string[])
                n375 = property on="DesignPatternList" class="LstBox (strict)"() -> ("Item Symbols"=w711:i32[])  [unwired: 2 in, 2 out]
                n376 = Index Array(array=w711, index=w704) -> (element=w710:i32)
                n377 = Equal?(x=w710, y=37) -> (x = y?=w707:bool)
                n378 = Index Array(array=w705, index=w704) -> (element=w703:string)
                n379 = case shown="True" w707 {
                  tunnel: w712 -> [w720 w741]
                  tunnel: w705 -> [_ w740]
                  tunnel: w704 -> [w719 w739]
                  tunnel: [w717 w735] -> w708
                  tunnel: [37 38] -> w706
                  tunnel: w703 -> [w721 _]
                  frame False {
                    # "Uncheck this any and other selected DP that is dependent on this DP"
                    n380 = Build Array(w719) -> (w718:i32[])
                    n381 = for {
                      tunnel: w721 -> [w727]
                      tunnel: w720 -> [w729] mode=indexing
                      shift-right: [w724] -> w717
                      shift-left: w718 -> [w725]
                      i -> [w723]
                      n382 = Unbundle(w729) -> ("DependenciesID"=w728:string[])
                      n383 = Search 1D Array(1D array=w728, element=w727) -> (index of element=w726:i32)  [unwired: 1 in]
                      n384 = case shown="0, Default" w726 {
                        tunnel: w725 -> [w732 w733]
                        tunnel: [w731 w733] -> w724
                        tunnel: w723 -> [w730 _]
                        frame 0, Default {
                          n385 = Build Array (concatenate)(w730, w732) -> (w731:i32[])
                        }
                        frame -1 {
                        }
                      }
                    }
                  }
                  frame True {
                    # "Check this Dp and all it's dependency DPs"
                    n386 = Index Array(array=w741, index=w739) -> (element=w738:cluster{"DependenciesID":string[]})
                    n387 = Unbundle(w738) -> ("DependenciesID"=w737:string[])
                    n388 = for {
                      tunnel: w740 -> [w744]
                      tunnel: w737 -> [w743] mode=indexing
                      tunnel: [w742] -> w736 mode=indexing
                      n389 = Search 1D Array(1D array=w744, element=w743) -> (index of element=w742:i32)  [unwired: 1 in]
                    }
                    n390 = Build Array (concatenate)(w736, w739) -> (w735:i32[])
                  }
                }
                n391 = for {
                  shift-right: [w748] -> w715
                  shift-left: w711 -> [w747]
                  tunnel: w708 -> [w746] mode=indexing
                  tunnel: w706 -> [w745]
                  n392 = in-place {
                    in-place-border: w745 -> [w749]
                    n393 = in-place-array #2(w747, w746) -> ()  [unwired: 1 out]
                    n394 = in-place-array #2(w749) -> (w748:i32[])  [unwired: 1 out]
                  }
                }
                n395 = property on="DesignPatternList" class="LstBox (strict)"("Item Symbols"=w715) -> ()  [unwired: 2 in, 2 out]
              }
              event "DesignPatternList": Mouse Down {
                n396 = event-data() -> ("CtlRef"=w753:refnum<vi>, "Coords"=w752:T30)  [unwired: 1 in]
                n397 = invoke class="LstBox (strict)" method="Point To Row"(reference=w753, "Point"=w752) -> ("Row"=w751:i32, "InGlyph"=w750:bool)  [unwired: 5 in, 5 out]
                n398 = case shown="True" w750 {
                  tunnel: w754 -> [_ w767]
                  tunnel: w751 -> [_ w757]
                  frame False {
                  }
                  frame True {
                    n399 = Unbundle By Name(w767) -> ("DpDependencies"=w766:cluster{"DependenciesID":string[]}[], "DPs"=w759:string[])
                    n400 = property on="DesignPatternList" class="LstBox (strict)"() -> ("Item Symbols"=w765:i32[])  [unwired: 2 in, 2 out]
                    n401 = Index Array(array=w759, index=w757) -> (element=w758:string)
                    n402 = Index Array(array=w765, index=w757) -> (element=w764:i32)
                    n403 = Equal?(x=w764, y=37) -> (x = y?=w761:bool)
                    n404 = case shown="True" w761 {
                      tunnel: w766 -> [w772 w793]
                      tunnel: w759 -> [_ w792]
                      tunnel: w757 -> [w771 w791]
                      tunnel: [w769 w787] -> w762
                      tunnel: [37 38] -> w760
                      tunnel: w758 -> [w773 _]
                      frame False {
                        # "Uncheck this any and other selected DP that is dependent on this DP"
                        n405 = Build Array(w771) -> (w770:i32[])
                        n406 = for {
                          tunnel: w773 -> [w779]
                          tunnel: w772 -> [w781] mode=indexing
                          shift-right: [w776] -> w769
                          shift-left: w770 -> [w777]
                          i -> [w775]
                          n407 = Unbundle(w781) -> ("DependenciesID"=w780:string[])
                          n408 = Search 1D Array(1D array=w780, element=w779) -> (index of element=w778:i32)  [unwired: 1 in]
                          n409 = case shown="0, Default" w778 {
                            tunnel: w777 -> [w784 w785]
                            tunnel: [w783 w785] -> w776
                            tunnel: w775 -> [w782 _]
                            frame 0, Default {
                              n410 = Build Array (concatenate)(w782, w784) -> (w783:i32[])
                            }
                            frame -1 {
                            }
                          }
                        }
                      }
                      frame True {
                        # "Check this Dp and all \nit's dependency DPs"
                        n411 = Index Array(array=w793, index=w791) -> (element=w790:cluster{"DependenciesID":string[]})
                        n412 = Unbundle(w790) -> ("DependenciesID"=w789:string[])
                        n413 = for {
                          tunnel: w792 -> [w796]
                          tunnel: w789 -> [w795] mode=indexing
                          tunnel: [w794] -> w788 mode=indexing
                          n414 = Search 1D Array(1D array=w796, element=w795) -> (index of element=w794:i32)  [unwired: 1 in]
                        }
                        n415 = Build Array (concatenate)(w788, w791) -> (w787:i32[])
                      }
                    }
                    n416 = for {
                      shift-right: [w800] -> w768
                      shift-left: w765 -> [w799]
                      tunnel: w762 -> [w798] mode=indexing
                      tunnel: w760 -> [w797]
                      n417 = in-place {
                        in-place-border: w797 -> [w801]
                        n418 = in-place-array #3(w799, w798) -> ()  [unwired: 1 out]
                        n419 = in-place-array #3(w801) -> (w800:i32[])  [unwired: 1 out]
                      }
                    }
                    n420 = property on="DesignPatternList" class="LstBox (strict)"("Item Symbols"=w768) -> ()  [unwired: 2 in, 2 out]
                  }
                }
              }
              event "_ClassName": Value Change {
                n421 = event-data() -> ("OldVal"=w807:string)  [unwired: 1 in]
                n422 = case shown="False" w803 {
                  tunnel: [w821 _] -> w802
                  frame False {
                    n423 = local read "_ClassFolderSuffix"() -> (w821:string)
                  }
                  frame True {
                  }
                }
                n424 = local read "_ClassFolder"() -> (w814:path)
                n425 = Concatenate Strings(w807, ".llb" ("t")) -> (w805:string)
                n426 = call <resource>:"GOOP300_RemoveUnwantedChars.vi"("StringIn"="_ClassName") -> ("StringOut"=w817:string)  [unwired: 10 in]
                n427 = Strip Path(path=w814) -> (stripped path=w815:path, name=w808:string)
                n428 = Concatenate Strings(w807, w802) -> (w816:string)
                n429 = local write "_ClassName"(w817) -> ()
                n430 = Equal?(x=w808, y=w816) -> (x = y?=w810:bool)
                n431 = Equal?(x=w808, y=w805) -> (x = y?=w809:bool)
                n432 = Or(x=w810, y=w809) -> (x .or. y?=w811:bool)
                n433 = Select(t=w815, s=w811, f=w814) -> (s? t:f=w813:path)
                n434 = local read "_UseLLB"() -> (w812:bool)
                n435 = case shown="Default" w817 {
                  selector: w817 -> [_ w827]
                  tunnel: [w822 w830] -> w820
                  tunnel: w802 -> [_ w825]
                  tunnel: w813 -> [w822 w828]
                  tunnel: w812 -> [_ w826]
                  frame "" {
                  }
                  frame Default {
                    n436 = Select(t=".llb", s=w826, f=w825) -> (s? t:f=w824:string)
                    n437 = Concatenate Strings(w827, w824) -> (w829:string)
                    n438 = Build Path(base path=w828, name or relative path=w829) -> (appended path=w830:path)
                  }
                }
                n439 = local write "_ClassFolder"(w820) -> ()
              }
              event "_SelectParentClass": Value Change {
                n440 = event-data() -> ()  [unwired: 1 in, 1 out]
                n441 = Unbundle By Name(w844) -> ("ClassPaths"=w835:path[], "DeriveFromClassRef"=w843:refnum<vi>, "ClassTags"=w831:string[], "BaseObjectTag"=w838:string)
                n442 = Not Equal?(x=w838, y="_SelectParentClass") -> (x != y?=w837:bool)
                n443 = for {
                  tunnel: w835 -> [w860] mode=indexing
                  tunnel: [w858] -> _ mode=indexing
                  n444 = Strip Path(path=w860) -> (name=w859:string)  [unwired: 1 out]
                  n445 = Match Pattern(string=w859, regular expression="\\2Elvclass$") -> (before substring=w858:string)  [unwired: 1 in, 3 out]
                }
                n446 = Close Reference(reference=w843) -> (error out=w842:errorcluster)  [unwired: 1 in]
                n447 = stacked-sequence {
                  tunnel: w842 -> [_]
                  tunnel: w835 -> [w861]
                  tunnel: [w861] -> w834
                  frame #0 {
                  }
                }
                n448 = Search 1D Array(1D array=w831, element="_SelectParentClass") -> (index of element=w832:i32)  [unwired: 1 in]
                n449 = Index Array(array=w834, index=w832) -> (element=w836:path)
                n450 = case shown="-1" w832 {
                  tunnel: w841 -> [w850 w855]
                  tunnel: [w849 w854] -> w840
                  tunnel: ["OpenDerivedBaseClass\nGetTemplates" "GetTemplates"] -> w839
                  tunnel: w837 -> [w847 _]
                  tunnel: w836 -> [w845 _]
                  frame 0, Default {
                    n451 = disable-structure shown="Disabled" {
                      disable-tunnel: [w852 _] -> w846
                      disable-tunnel: w845 -> [w851 _]
                      frame Disabled {
                        n452 = call <resource>:"GDSLvClass_OpenClass.vi"("ClassToOpen"=w851) -> ("LVClass.Open"=w852:refnum<vi>)  [unwired: 17 in, 1 out]
                      }
                      frame Enabled {
                      }
                    }
                    n453 = Bundle By Name(cluster=w850, "Derived"=w847, "DeriveFromClass"=w845, "DeriveFromClassRef"=w846) -> (w849:T13)
                  }
                  frame -1 {
                    n454 = Bundle By Name(cluster=w855, "Derived"=FALSE) -> (w854:T13)
                  }
                }
              }
              event "InterfaceFilter": Value Change {
                n455 = event-data() -> ()  [unwired: 1 in, 6 out]
              }
              event "ParentClassFilter": Value Change {
                n456 = event-data() -> ()  [unwired: 1 in, 6 out]
              }
              event "_SelectInterfaceClass": Value Change {
                n457 = event-data() -> ()  [unwired: 1 in, 6 out]
                n458 = Unbundle By Name(w871) -> ("InterfacesInList"=w872:path[])
                n459 = for {
                  tunnel: "_SelectInterfaceClass" -> [w875] mode=indexing
                  tunnel: w872 -> [w876]
                  tunnel: [w874] -> w873 mode=indexing
                  n460 = Index Array(array=w876, index=w875) -> (element=w874:path)
                }
                n461 = Empty Array?(array="_SelectInterfaceClass") -> (empty?=w867:bool)
                n462 = call <resource>:"GDSControl_Disable.vi"("Disasble(True)"=w867) -> ("Enable Property"=w866:T19)  [unwired: 10 in]
                n463 = property on="CreateInterfaceMethods" class="Enum (strict)"("DisabledEnum"=w866) -> ()  [unwired: 2 in, 2 out]
                n464 = Bundle By Name(cluster=w870, "ParentInterfaces"=w873) -> (w869:T13)
              }
              event "_UseLLB": Value Change {
                n465 = event-data() -> ()  [unwired: 1 in, 2 out]
                n466 = Select(t=u8 2 ("Disabled"), s="_UseLLB", f=u8 0 ("Disabled")) -> (s? t:f=w881:u8)
                n467 = property on="_ClassName" class="Str"() -> ("Value"=w878:string)  [unwired: 2 in, 2 out]
                n468 = property on="_ClassFolderSuffix" class="Str"("Disabled"=w881) -> ()  [unwired: 2 in, 2 out]
                n469 = property on="_ClassName" class="Str"("Val(Sgnl)"=w878) -> ()  [unwired: 2 in, 2 out]
              }
              event "_ShowContextHelp": Value Change {
                n470 = event-data() -> ("NewVal"=w884:bool)  [unwired: 1 in]
                n471 = Control Help Window(1:w884) -> ()  [unwired: 1 in]
              }
              event "_ClassFolderSuffix", "TriggerSuffixChange": Value Change {
                n472 = event-data() -> ("OldVal"=w888:string)  [unwired: 1 in, 2 out]
                n473 = local read "_ClassFolder"() -> (w902:path)
                n474 = call <resource>:"GOOP300_RemoveUnwantedChars.vi"("StringIn"="_ClassFolderSuffix") -> ("StringOut"=w889:string)  [unwired: 10 in]
                n475 = local write "_ClassFolderSuffix"(w889) -> ()
                n476 = Strip Path(path=w902) -> (stripped path=w897:path, name=w899:string)
                n477 = Select(t="", s=w892, f=w889) -> (s? t:f=w891:string)
                n478 = Build Array(w889, w888) -> (w887:string[])
                n479 = local read "_ClassName"() -> (w894:string)
                n480 = for {
                  tunnel: w887 -> [w904] mode=indexing
                  shift-right: [w905] -> w898
                  shift-left: w899 -> [w908]
                  n481 = Concatenate Strings(w904, "$" ("string")) -> (w907:string)
                  n482 = Match Pattern(string=w908, regular expression=w907) -> (before substring=w905:string)  [unwired: 1 in, 3 out]
                }
                n483 = Empty String/Path?(string/path=w894) -> (empty?=w893:bool)
                n484 = Concatenate Strings(w898, w891) -> (w896:string)
                n485 = Build Path(base path=w897, name or relative path=w896) -> (appended path=w895:path)
                n486 = case shown="False" w893 {
                  tunnel: w895 -> [w909 _]
                  frame False {
                    n487 = local write "_ClassFolder"(w909) -> ()
                  }
                  frame True {
                  }
                }
              }
              event "_ClassFolder": Value Change {
                n488 = event-data() -> ()  [unwired: 1 in, 2 out]
                n489 = Strip Path(path="_ClassFolder") -> ()  [unwired: 2 out]
                n490 = property on="_ClassName" class="Str"() -> ("Value"=w911:string)  [unwired: 2 in, 2 out]
                n491 = property on="_ClassName" class="Str"("Val(Sgnl)"=w911) -> ()  [unwired: 2 in, 2 out]
              }
            }
            n492 = Bundle By Name(cluster=w522, "Cancel"=w540) -> (w538:T13)
          }
          frame "OpenDerivedBaseClass" {
            n493 = Unbundle By Name(w914) -> ("DeriveFromClass"=w916:path)
            n494 = call <resource>:"GDSLvClass_OpenClass.vi"("ClassToOpen"=w916) -> ("LVClass.Open"=w917:refnum<vi>)  [unwired: 17 in, 1 out]
            n495 = Bundle By Name(cluster=w914, "DeriveFromClassRef"=w917) -> (w915:T13)
          }
          frame "UpdateTemplates" {
            n496 = call-dynamic "GetProviderName.vi"("ClassWriterNative in"=w921) -> ("ShortName(Could be used in for INI Sections)"=w920:string)  [unwired: 14 in, 4 out]
            n497 = Unbundle By Name(w928) -> ("Templates"=w925:T10[], "ClassTemplateIndex"=w927:i32[])
            n498 = local read "_ClassType"() -> (w926:i32)
            n499 = Index Array(array=w927, index=w926) -> (element=w924:i32)
            n500 = Index Array(array=w925, index=w924) -> (element=w923:T10)
            n501 = Unbundle By Name(w923) -> ("TemplateIdName"=w922:string)
            n502 = call <resource>:"DialogCreateClass_FilterAndOrderClassTemplates.vi"("ProviderShortName"=w920, "AllTemplatesForThisProvider/InheritanceType(Base/Sub)"=w925) -> ("NewOrderIndex"=w942:i32[], "FilteredTemplates"=w929:T10[])  [unwired: 7 in, 1 out]
            n503 = for {
              tunnel: w929 -> [w951] mode=indexing
              tunnel: [w950] -> w941 mode=indexing
              tunnel: [w949] -> w940 mode=indexing
              tunnel: [w948] -> w938 mode=indexing
              tunnel: [w947] -> w936 mode=indexing
              n504 = Unbundle(w951) -> ("TemplateIdName"=w949:string, "TemplateUserDialogName"=w950:string, "ClassSuffix"=w948:string, "LvLibTemplate"=w947:bool)  [unwired: 4 out]
            }
            n505 = Bundle By Name(cluster=w928, "ClassTemplateIndex"=w942) -> (w943:T13)
            n506 = Search 1D Array(1D array=w940, element=w922) -> (index of element=w939:i32)  [unwired: 1 in]
            n507 = Max & Min(x=w939, y=0 ("Class Type")) -> (max(x,y)=w935:i32)  [unwired: 1 out]
            n508 = Index Array(array=w938, index=w935) -> (element=w937:string)
            n509 = Index Array(array=w936, index=w935) -> (element=w934:bool)
            n510 = property on="_ClassType" class="LstBox (strict)"("Item Names"=w941, "Val(Sgnl)"=w935) -> ()  [unwired: 2 in, 2 out]
            n511 = case shown="Default" w937 {
              selector: w937 -> [_ w946]
              frame "" {
              }
              frame Default {
                n512 = property on="_ClassFolderSuffix" class="Str"("Val(Sgnl)"=w946) -> ()  [unwired: 2 in, 2 out]
              }
            }
            n513 = Select(t="Library folder (The lvlib file will be saved in this directory)", s=w934, f=w930) -> (s? t:f=w933:string)
            n514 = property on="_ClassFolder" class="Path"("Caption.Text"=w933) -> ()  [unwired: 2 in, 2 out]
          }
          frame "GetDesignPatterns" {
            w953 = string[] []
            n515 = Unbundle By Name(w957) -> ("ClassProviderName"=w968:string, "ClassTemplateUsed"=w967:string)  [unwired: 1 out]
            n516 = call <resource>:"BaseProvider_DesignPattern_GetPatterns.vi"("FilterOnProviders(Ignored If Empty)"=w968, "FilterOnTemplate(Ignored If Empty)"=w967, "error in (no error)"=w966) -> ("DesignPatterns"=w964:T31[], "error out"=w965:errorcluster)  [unwired: 15 in]
            n517 = for {
              tunnel: w964 -> [w982] mode=indexing
              shift-right: [w979] -> w958
              shift-left: w953 -> [w978]
              shift-right: [w977] -> w960
              shift-left: w953 -> [w976]
              shift-right: [w975] -> w962
              shift-left: i32[] [] -> [w974]
              shift-right: [w972] -> w954
              shift-left: cluster{"DependenciesID":string[]}[] [] -> [w973]
              shift-right: [w971] -> w952
              shift-left: w953 -> [w970]
              n518 = Unbundle By Name(w982) -> ("Type"=w980:string, "Patterns"=w981:T32)
              n519 = for {
                tunnel: w981 -> [w1007] mode=indexing
                tunnel: w980 -> [w1006]
                shift-right: [w1002] -> w979
                shift-left: w978 -> [w1001]
                shift-right: [w998] -> w977
                shift-left: w976 -> [w999]
                shift-right: [w995] -> w975
                shift-left: w974 -> [w994]
                shift-right: [w985] -> w972
                shift-left: w973 -> [w984]
                shift-right: [w988] -> w971
                shift-left: w970 -> [w987]
                n520 = Unbundle By Name(w1007) -> ("ID"=w989:string, "Name"=w1005:string, "Desc"=w991:string, "Version"=w1003:string, "DependenciesID"=w983:string[])  [unwired: 1 out]
                n521 = Array Size(array=w983) -> (size(s)=w992:i32)
                n522 = case shown="1.." w992 {
                  tunnel: ["" w1010] -> w990
                  tunnel: w983 -> [_ w1009]
                  frame 0, Default {
                  }
                  frame 1.. {
                    n523 = Array To Spreadsheet String(delimiter (Tab)=", ", array=w1009, 3:"%s" ("format string")) -> (spreadsheet string=w1011:string)
                    n524 = Format Into String(format string="\nDependencies: %s", w1011) -> (resulting string=w1010:string)  [unwired: 2 in, 1 out]
                  }
                }
                n525 = Format Into String(format string="%s : %s", w1006, w1005) -> (resulting string=w996:string)  [unwired: 2 in, 1 out]
                n526 = Bundle("DependenciesID"=w983) -> (w986:cluster{"DependenciesID":string[]})  [unwired: 1 in]
                n527 = Format Into String(format string="%s%s\n[%s, version: %s]", w991, w990, w989, w1003) -> (resulting string=w1000:string)  [unwired: 2 in, 1 out]
                n528 = Build Array (concatenate)(w984, w986) -> (w985:cluster{"DependenciesID":string[]}[])
                n529 = Build Array (concatenate)(w987, w989) -> (w988:string[])
                n530 = Build Array (concatenate)(w999, w996) -> (w998:string[])
                n531 = Build Array (concatenate)(w1001, w1000) -> (w1002:string[])
                n532 = Build Array (concatenate)(w994, 37) -> (w995:i32[])
              }
            }
            n533 = property on="DesignPatternList" class="LstBox (strict)"("Item Names"=w960, "Item Symbols"=w962, "Value"=-1 ("Design Patterns"), "SelColor"=u32 14342874) -> ()  [unwired: 2 in, 2 out]
            n534 = Bundle By Name(cluster=w957, "DPs"=w952, "DPDescriptions"=w958, "DpDependencies"=w954) -> (w956:T13)
          }
          frame "GetClassTemplateToUse" {
            n535 = Unbundle By Name(w1018) -> ("ClassPaths"=w1022:path[], "ClassTags"=w1023:string[], "BaseClasses"=w1043:path[])  [unwired: 1 out]
            n536 = Unbundle By Name(w1018) -> ("Templates"=w1041:T10[], "DesignPatternsVisible"=w1037:bool)
            n537 = local read "_SelectParentClass"() -> (w1024:string)
            n538 = Unbundle By Name(w1018) -> ("Templates"=w1030:T10[], "ClassTemplateIndex"=w1021:i32[])
            n539 = local read "_ClassType"() -> (w1020:i32)
            n540 = for {
              tunnel: w1041 -> [w1085] mode=indexing
              tunnel: [w1084] -> w1040 mode=indexing
              n541 = Unbundle By Name(w1085) -> ("TemplateIdName"=w1084:string)  [unwired: 1 out]
            }
            n542 = disable-structure shown="Enabled" {
              disable-tunnel: w1043 -> [w1052 _]
              disable-tunnel: [w1051 w1059] -> w1042
              disable-tunnel: w1024 -> [w1047 w1062]
              disable-tunnel: w1023 -> [_ w1063]
              disable-tunnel: w1022 -> [_ w1061]
              frame Disabled {
                n543 = for {
                  tunnel: w1052 -> [w1058] mode=indexing
                  tunnel: [w1055] -> w1054 mode=indexing
                  n544 = Strip Path(path=w1058) -> (name=w1057:string)  [unwired: 1 out]
                  n545 = Match Pattern(string=w1057, regular expression="\\2E[Ll][Vv][Cc][Ll][Aa][Ss][Ss]$") -> (before substring=w1055:string)  [unwired: 1 in, 3 out]
                }
                n546 = To Lower Case(string=w1054) -> (all lower case string=w1053:string[])
                n547 = Match Pattern(string=w1047, regular expression="\\2E[Ll][Vv][Cc][Ll][Aa][Ss][Ss]$") -> (before substring=w1046:string)  [unwired: 1 in, 3 out]
                n548 = To Lower Case(string=w1046) -> (all lower case string=w1049:string)
                n549 = Search 1D Array(1D array=w1053, element=w1049) -> (index of element=w1050:i32)  [unwired: 1 in]
                n550 = Index Array(array=w1052, index=w1050) -> (element=w1051:path)
              }
              frame Enabled {
                n551 = Search 1D Array(1D array=w1063, element=w1062) -> (index of element=w1060:i32)  [unwired: 1 in]
                n552 = Index Array(array=w1061, index=w1060) -> (element=w1059:path)
              }
            }
            n553 = case shown="True" w1037 {
              tunnel: w1018 -> [_ w1081]
              tunnel: [_ w1076] -> w1038
              frame False {
              }
              frame True {
                n554 = property on="DesignPatternList" class="LstBox (strict)"() -> ("Item Symbols"=w1080:i32[])  [unwired: 2 in, 2 out]
                n555 = Unbundle By Name(w1081) -> ("DPs"=w1077:string[])
                n556 = Equal?(x=w1080, y=38) -> (x = y?=w1078:bool[])
                n557 = for {
                  tunnel: w1078 -> [w1082] mode=indexing
                  tunnel: w1077 -> [w1083] mode=indexing
                  tunnel: [w1083] -> w1076 mode=indexing if=w1082
                }
              }
            }
            n558 = Index Array(array=w1021, index=w1020) -> (element=w1019:i32)
            n559 = Index Array(array=w1030, index=w1019) -> (element=w1029:T10)
            n560 = Unbundle By Name(w1029) -> ("ClassSuffix"=w1026:string)
            n561 = Unbundle By Name(w1018) -> ("ClassTemplateIndex"=w1017:i32[])
            n562 = property on="_ClassType" class="LstBox (strict)"() -> ("Value"=w1016:i32)  [unwired: 2 in, 2 out]
            n563 = Empty String/Path?(string/path=w1026) -> (empty?=w1027:bool)
            n564 = Index Array(array=w1017, index=w1016) -> (element=w1015:i32)
            n565 = local read "_ClassFolderSuffix"() -> (w1031:string)
            n566 = Index Array(array=w1040, index=w1015) -> (element=w1039:string)
            n567 = call <resource>:"BaseProvider_IniFileSettings.vi"("Action"=enum16{"Read", "Load", "Save"}."Read") -> ("IniFileSettings"=w1032:T24)  [unwired: 17 in, 1 out]
            n568 = Unbundle By Name(w1032) -> ("ClassFolderSuffix"=w1033:string)
            n569 = Not Equal?(x=w1033, y=w1031) -> (x != y?=w1028:bool)
            n570 = And(x=w1028, y=w1027) -> (x .and. y?=w1025:bool)
            n571 = case shown="True" w1025 {
              tunnel: w1036 -> [w1064 w1068]
              tunnel: [w1064 w1067] -> w1035
              tunnel: w1032 -> [_ w1066]
              tunnel: w1031 -> [_ w1065]
              frame False {
              }
              frame True {
                n572 = case shown="Default" w1065 {
                  selector: w1065 -> [_ w1070]
                  tunnel: w1068 -> [w1069 w1074]
                  tunnel: [w1069 w1073] -> w1067
                  tunnel: w1066 -> [_ w1072]
                  frame "_Actor", "_Msg" {
                  }
                  frame Default {
                    n573 = Bundle By Name(cluster=w1072, "ClassFolderSuffix"=w1070) -> (w1071:T24)
                    n574 = call <resource>:"BaseProvider_IniFileSettings.vi"("IniFileSettings"=w1071, "error in (no error)"=w1074, "Action"=enum16{"Read", "Load", "Save"}."Save") -> ("error out"=w1073:errorcluster)  [unwired: 15 in, 1 out]
                  }
                }
              }
            }
            n575 = Bundle By Name(cluster=w1018, "ClassType(Template)"=w1039, "DPs"=w1038, "BaseClassToUse"=w1042) -> (w1045:T13)
          }
          frame "GetInterfaceSettings" {
            n576 = local read "_SelectInterfaceClass"() -> (w1097:i32[])
            n577 = property on="_SelectInterfaceClass" class="MCListbox (strict)"() -> ("ItemNames"=w1100:string[][])  [unwired: 2 in, 2 out]
            n578 = Unbundle By Name(w1096) -> ("InterfaceInfo"=w1094:T11[])
            n579 = Index Array(array=w1100, index (col)=0 ("disabled index (col)")) -> (element=w1098:string[])  [unwired: 1 in]
            n580 = for {
              tunnel: w1094 -> [w1110] mode=indexing
              tunnel: [w1109] -> w1095 mode=indexing
              n581 = Unbundle By Name(w1110) -> ("Name(Short if no Conflicts)"=w1109:string)
            }
            n582 = for {
              tunnel: w1098 -> [w1118]
              tunnel: w1097 -> [w1117] mode=indexing
              tunnel: w1095 -> [w1116]
              tunnel: w1094 -> [w1114]
              tunnel: [w1112] -> w1086 mode=indexing
              tunnel: [w1111] -> w1087 mode=indexing
              n583 = Index Array(array=w1118, index=w1117) -> (element=w1115:string)
              n584 = Search 1D Array(1D array=w1116, element=w1115) -> (index of element=w1113:i32)  [unwired: 1 in]
              n585 = Index Array(array=w1114, index=w1113) -> (element=w1111:T11)
              n586 = Unbundle By Name(w1111) -> ("Path"=w1112:path)
            }
            n587 = local read "CreateInterfaceMethods"() -> (w1089:T4)
            n588 = case shown="\"Create all interface methods\"" w1089 {
              tunnel: [_ w1105 w1108] -> w1088
              tunnel: w1087 -> [_ w1104 w1107]
              frame Default {
              }
              frame "Create all interface methods" {
                n589 = Array Size(array=w1104) -> (size(s)=w1106:i32)
                n590 = Initialize Array(cluster{"Methods":string[]} {"Methods"=[]} ("Methods"), w1106) -> (w1105:cluster{"Methods":string[]}[])
              }
              frame "Create some interface methods" {
                n591 = call <resource>:"SelectMethodsOfInterfaces.vi"("InterfacePath"=w1107) -> ("MethodsPerInterface(Empty=>All)"=w1108:cluster{"Methods":string[]}[])  [unwired: 9 in, 1 out]
              }
            }
            n592 = Greater Or Equal?(x=w1089, y=T4."Create some interface methods") -> (x >= y?=w1090:bool)
            n593 = Bundle By Name(cluster=T5 {"InterfacePath"=[], "CreateMethods"=FALSE, "MethodsPerInterface(Empty=>All)"=[]} ("InterfaceToImplement"), "InterfacePath"=w1086, "CreateMethods"=w1090, "MethodsPerInterface(Empty=>All)"=w1088) -> (→"InterfaceToImplement":T5)
          }
          frame "Error", Default {
          }
          frame "Exit" {
          }
        }
        n594 = call <vilib>:"Clear Errors.vi"("error in (no error)"=w62) -> ()  [unwired: 5 in, 2 out]
      }
      n595 = call <vilib>:"Clear Errors.vi"("error in (no error)"=w45) -> ("error out"=w44:errorcluster)  [unwired: 5 in, 1 out]
      n596 = call <resource>:"GDSString_AddStatesToQueue.vi"() -> ()  [unwired: 15 in, 1 out]
      n597 = property on="_ClassFolder" class="Path"(error in=w44, "Caption.Text"=w48) -> ()  [unwired: 1 in, 2 out]
    }
    frame Error {
    }
  }
  "Reference out" <- w40
  "error out" <- w42
  n598 = Generate User Event(user event=w20, event data cluster="Stop" ("Stop")) -> (user event out=w22:refnum<user-event>)  [unwired: 2 in, 1 out]
  n599 = Destroy User Event(user event=w22) -> ()  [unwired: 1 in, 1 out]
  n600 = Get Date/Time In Seconds() -> ()  [unwired: 1 out]
  n601 = stacked-sequence {
    tunnel: w39 -> [w1131]
    tunnel: [w1146] -> w38
    tunnel: [w1145] -> w37
    tunnel: [w1141] -> w34
    tunnel: [w1144] -> w36
    tunnel: [w1143] -> w35
    tunnel: [w1142] -> w33
    tunnel: [w1140] -> _
    tunnel: "ProjectItem Refnum" -> [w1137]
    tunnel: w29 -> [w1136]
    tunnel: [w1134] -> w28
    tunnel: [w1133] -> w27
    tunnel: [w1132] -> w26
    tunnel: [w1130] -> w7
    frame #0 {
      n602 = Unbundle By Name(w1131) -> ("DesignPatternsVisible"=w1135:bool, "Cancel"=w1146:bool, "BaseClassToUse"=w1141:path, "ClassType(Template)"=w1142:string, "DeriveFromClassRef"=w1139:refnum<vi>)
      n603 = case shown="True" w1135 {
        tunnel: w1136 -> [_ w1147]
        frame False {
        }
        frame True {
          n604 = property class="VI"() -> ("Front Panel.PanelBounds"=w1149:T9)  [unwired: 2 in, 2 out]
          n605 = Subtract(x=w1149, y=w1147) -> (x-y=w1148:T9)
          n606 = property class="VI"("Front Panel.PanelBounds"=w1148) -> ()  [unwired: 2 in, 2 out]
        }
      }
      n607 = local read "_ClassFolder"() -> (w1145:path)
      n608 = local read "_ClassName"() -> (w1144:string)
      n609 = local read "_ClassDescription"() -> (w1143:string)
      n610 = local read "_ClassFolderSuffix"() -> (w1132:string)
      n611 = Unbundle By Name(w1131) -> ("ChangeProviderTo"=w1133:string)
      n612 = Unbundle By Name(w1131) -> ("ParentInterfaces"=w1130:path[])
      n613 = Not Equal?(x=w1139, y=w1137) -> (x != y?=w1138:bool)
      n614 = Unbundle By Name(w1131) -> ("DPs"=w1134:string[])
      n615 = case shown="True" w1138 {
        tunnel: [_ w1151] -> w1140
        tunnel: w1139 -> [_ w1150]
        frame False {
        }
        frame True {
          n616 = Close Reference(reference=w1150) -> (error out=w1151:errorcluster)  [unwired: 1 in]
        }
      }
    }
  }
  "Cancelled" <- w38
  "DesignPatternsToAddAfterCreation" <- w28
  "ChangeProviderRequested" <- w27
  n617 = Bundle By Name(cluster=T6 {"ClassName"="", "ClassFolder"=path "", "ClassDescription"="", "ClassTemplateOptions"="", "BaseClass(ProjectStringPath or LvClassFilePath)"=variant, "ExtraCreateParameters"=variant, "FolderSuffix"="", "ParentInterfaces"=[]} ("CreateClassData"), "ClassFolder"=w37, "ClassName"=w36, "ClassDescription"=w35, "BaseClass(ProjectStringPath or LvClassFilePath)"=w34, "ClassTemplateOptions"=w33, "FolderSuffix"=w26, "ParentInterfaces"=w7) -> (→"CreateClassData":T6)
